vi "步进电机 - MO1.vi"() -> ()   [LabVIEW 2026, in "UI-步进.lvlib"]
doc: "本范例执行串口读写操作。串口设置的参数必须匹配连接仪器或设备的参数。“VISA配置串口”VI可设置配置参数。前面板显示的控件可用于配置基本参数，如波特率、数据位和校验。VI会将VISA资源名称传递至其他VI以便执行相关操作。“VISA写入”函数将发送一个命令至串行设备，“VISA读取”函数将返回基于该命令的数据。“VISA关闭”函数可关闭该串行设备的引用。关闭引用十分重要，否则可能导致无法通过该端口进行进一步通信。"
uses:
  Data ColndSave/Supports/Time and Data.ctl
  Supports/Sample Settings.ctl
  Supports/Repeat Steps.ctl
  <userlib>/_NEVSTOP/Communicable State Machine(CSM)/_Polymophic/CSM - Filter Duplicated Lines.vi
  b0ea00e1-49fa-42d0-971a-8e9f2f400525.vi
  20f4c7ca-4433-4752-8a12-caedff3309a5.vi
  a83f89c7-cc94-454f-8c22-caf8203e03ac.vi
  b673ad46-ecaf-4cfd-8bbb-6ae2088f5605.vi
  2e9f0e78-498b-41e3-86b1-c1255401f045.vi
  04a4e073-6b30-45d7-bb50-3b2b3a136a6d.vi
  2a4e068b-7d24-4fa7-ac03-c345972a0de1.vi
  44b8d297-727d-4724-bbbb-13bdb1641d5d.vi
  723f4e3d-5d0c-4f32-90dc-14f06c7549ca.vi
  796b8098-58f3-468a-8e00-fd722edcd372.vi
  f0ef90a9-37fd-4693-8a17-3839f28c21af.vi
  f65ec2b2-16c2-4de3-b539-835afd05168c.vi
  fd098784-0da8-4741-84dc-d815f177a802.vi
  <userlib>/_NEVSTOP/Communicable State Machine(CSM)/_Polymophic/CSM - Replace Marks in Messages.vi
  990eb54c-669a-44f1-af6b-0d611d3b61bb.vi
  2b2daabb-4cfa-4505-9e37-d62c08413a28.vi
  9c881153-a381-4589-a185-2ba02b3623cc.vi
  a1f5b737-46a0-46ad-8ba4-fb05ffa8a237.vi
  d5c603ec-7b80-4271-a83a-f9475fd1a065.vi
  c59def73-e1a7-4980-a83b-4e794f8740d4.vi
  95a76b64-0183-4b9d-a020-bf71b96b4595.vi
  12ea21cb-d699-47f4-8962-41d5d90be2ef.vi
  666677ec-4a5d-482c-b398-180d4b47e7ed.vi
  494b3fb5-273a-41a7-af20-8ee63da9d16f.vi
  0af2ad88-edd2-4f06-96cf-8fa513af6a10.vi
  2532b81a-ef6f-4dde-8bfe-c4d2e445e585.vi
  41f7d585-ae95-49ce-8fbc-6366eab20bab.vi
  57b87adc-c73b-462d-8ae1-05c1c70c80b4.vi
  b9a08e84-7226-4261-ac85-d69acd1971d6.vi
  <userlib>/_NEVSTOP/Communicable State Machine(CSM)/AdvanceAPI/CSM - Compact Multiple States.vi
  <userlib>/_NEVSTOP/Communicable State Machine(CSM)/AdvanceAPI/CSM - Break Down Multiple States String.vi
  <userlib>/_NEVSTOP/Communicable State Machine(CSM)/_Shared/Remove Comments from Single-line.vi
  <userlib>/_NEVSTOP/Communicable State Machine(CSM)/_Shared/Split Single-line Message.vi
  <userlib>/_NEVSTOP/Communicable State Machine(CSM)/_Shared/Trim Single-line Text.vi
  <userlib>/_NEVSTOP/Communicable State Machine(CSM)/AdvanceAPI/CSM - Revert Arguments-Safe String.vi
  <userlib>/_NEVSTOP/Communicable State Machine(CSM)/AdvanceAPI/CSM - Make String Arguments Safe.vi
  723f4e3d-5d0c-4f32-90dc-14f06c7549ca.vi/99de0c97-112a-4c86-9094-c187659127e1.vi
  <userlib>/_NEVSTOP/Communicable State Machine(CSM)/Utility/Build Error Cluster.vi
  796b8098-58f3-468a-8e00-fd722edcd372.vi/99de0c97-112a-4c86-9094-c187659127e1.vi
  f65ec2b2-16c2-4de3-b539-835afd05168c.vi/99de0c97-112a-4c86-9094-c187659127e1.vi
  fd098784-0da8-4741-84dc-d815f177a802.vi/99de0c97-112a-4c86-9094-c187659127e1.vi
  2532b81a-ef6f-4dde-8bfe-c4d2e445e585.vi/b09b9099-6be0-413b-8afc-4908471460c3.vi
  <userlib>/_NEVSTOP/Communicable State Machine(CSM)/addons/INI-Static-Variable-Support/_Support/FlagInstance-CSMINIVariable.vi
  b9a08e84-7226-4261-ac85-d69acd1971d6.vi/99de0c97-112a-4c86-9094-c187659127e1.vi
  <vilib>/Utility/error.llb/Trim Whitespace.vi
  <vilib>/Utility/error.llb/Trim Whitespace (string).vi
  <userlib>/_NEVSTOP/Communicable State Machine(CSM)/AdvanceAPI/CSM - Keywords.vi
  <userlib>/_NEVSTOP/Communicable State Machine(CSM)/_Support/ChangeFlag/ChangeFlag-Read.vi
  <vilib>/Utility/error.llb/Trim Whitespace One-Sided.vi
  <userlib>/_NEVSTOP/Communicable State Machine(CSM)/addons/INI-Static-Variable-Support/_Support/instances/_CSM - Read File Logger Configuration - v1.0.vi
  <vilib>/Utility/Data Type/Get Type Information.vi
  <userlib>/_NEVSTOP/Communicable State Machine(CSM)/addons/API-String-Arugments-Support/_Support/Data To SingleElementsArray_csm.vi
  <userlib>/_NEVSTOP/Communicable State Machine(CSM)/addons/API-String-Arugments-Support/_Support/Data To API String Arguments.vi
  <userlib>/_NEVSTOP/Communicable State Machine(CSM)/addons/INI-Static-Variable-Support/_Support/Parse Used Session and Name.vi
  <userlib>/_NEVSTOP/Communicable State Machine(CSM)/addons/INI-Static-Variable-Support/_Support/INI-FGV(lvlibp).vi
  <userlib>/_NEVSTOP/Communicable State Machine(CSM)/addons/INI-Static-Variable-Support/_Support/Populate String with INI Variable.vi
  <userlib>/_NEVSTOP/Communicable State Machine(CSM)/addons/API-String-Arugments-Support/_Support/Convert API String Arguments to Data(variant).vi
  <userlib>/_NEVSTOP/Communicable State Machine(CSM)/addons/API-String-Arugments-Support/_Support/SingleElementsArray To Data_csm.vi
  <userlib>/_NEVSTOP/Communicable State Machine(CSM)/addons/MassData-Parameter/_support/FGV-MassData(lvlibp).vi
  <vilib>/Instr/_visa.llb/VISA Configure Serial Port (Instr).vi
  <userlib>/_NEVSTOP/Communicable State Machine(CSM)/_Support/ChangeFlag/ChangeFlagDB.vi
  <userlib>/_NEVSTOP/Communicable State Machine(CSM)/Communicable State Machine.lvlib
  <userlib>/_NEVSTOP/Communicable State Machine(CSM)/addons/INI-Static-Variable-Support/INI-Static-Variable-Support.lvlib
  <userlib>/_NEVSTOP/Communicable State Machine(CSM)/addons/MassData-Parameter/CSM MassData Parameter Support.lvlib
  <userlib>/_NEVSTOP/Communicable State Machine(CSM)/addons/Watchdog/CSM Watchdog.lvlib
  <userlib>/_NEVSTOP/Communicable State Machine(CSM)/addons/Logger/CSM File Logger.lvlib
  Logging/Logging.lvlib
  Acquisition/Acquisition.lvlib
  Data ColndSave/Data Collection and Save.lvlib
  Repeat/Repeat.lvlib
panel:
  in  "步进电机显示":enum32{"步进电机", "循环功能", "联动功能", "Status"}(tab)
  in  "一键回原点":bool
  out "设置/读取报错":bool
  out "运行状态":bool
  in  "行程":i32 max=10 step=1
  in  "停止运行":bool
  in  "暂停":bool
  in  "速度(r/min)":i32=70 max=10 step=1
  in  "运行":bool
  in  "脱机使能":bool
  in  "加减速系数(0-10)":u8 max=10 step=1
  in  "运行单位":enum32{"脉冲", "圈数", "角度"}(radio)
  in  "电机开关":bool
  in  "步进电机串口":refnum<visa-resource-name>="COM4"
  out "步进电机位置":waveform(dbl)(graph)
  in  "运行方向":bool
  in  "CSM Name":string="MO1"
  in  "Interval(s)":dbl=0.5
  in  "电机循环":bool
  out "Error Occurred":errorcluster caption="步进电机-错误输出"
  in  "子程序？":bool
  out "State History":string
  in  "停止":bool
  # "电机连接"
  # "运行设置"
  # "基础功能"
  # "运行控制"
  # "状态显示"
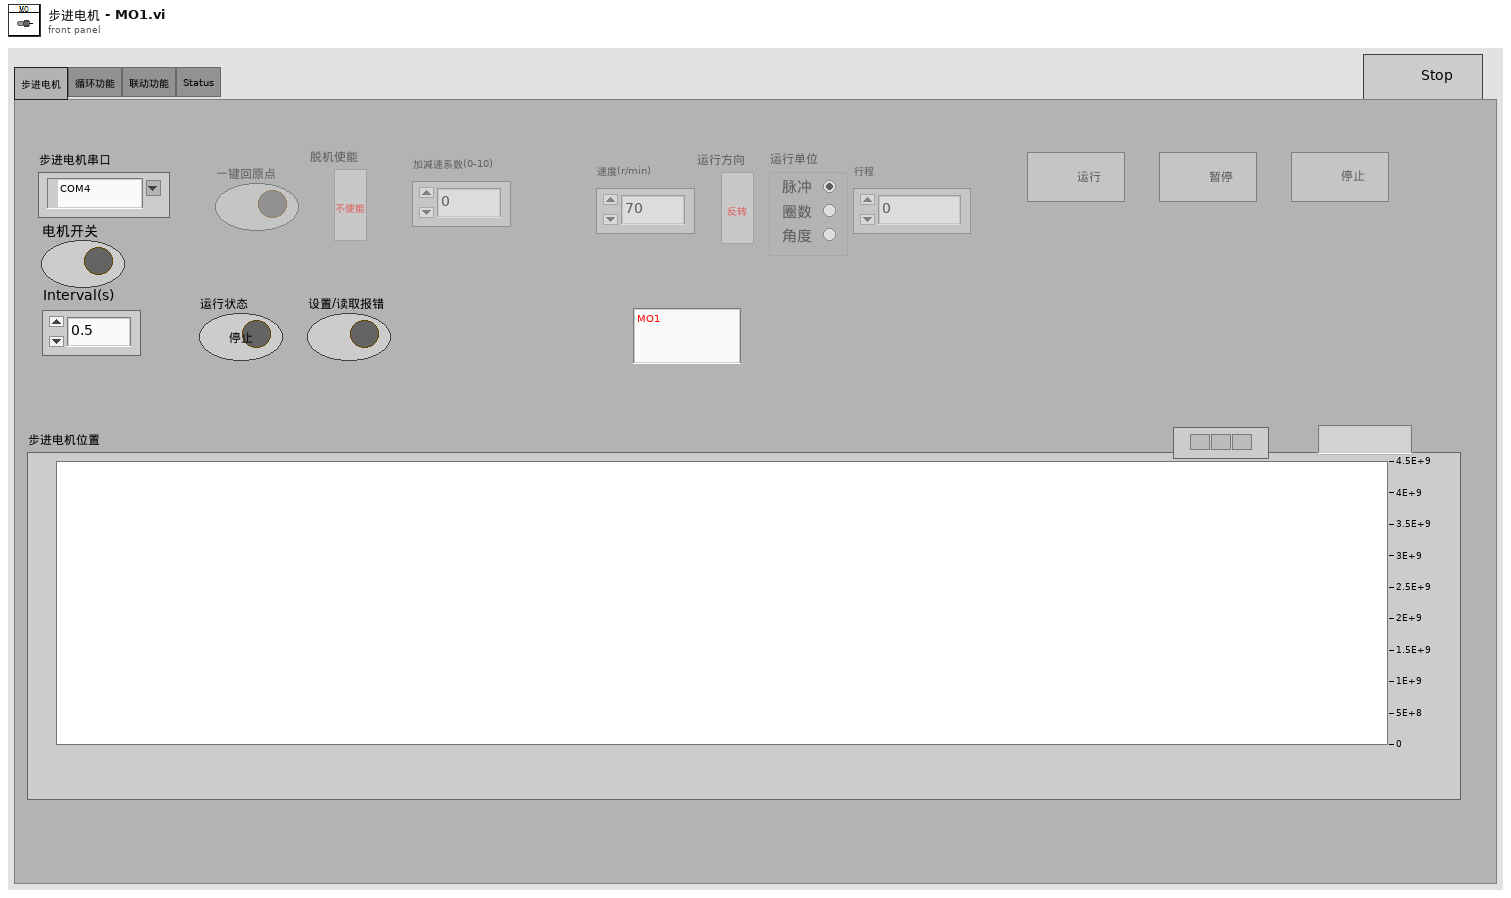
[diagram p1: front panel]
types:
  T1 = cluster{"Enable":bool, "Limit":cluster{"FileSize":i64, "FileNum":i32}, "Timestamp.Format":string, "AutoExit":bool}
  T2 = enum32{"Invalid", "Standard", "Closed", "Hidden", "Minimized", "Maximized"}
  T3 = enum32{"invalid app kind", "Development System", "Run Time System", "Student Edition", "Embedded LabVIEW", "Evaluation", "Custom"}
  T4 = cluster{"波特率":u32, "数据位":u16, "校验":enum16{"None", "Odd", "Even", "Mark", "Space"}, "停止位":u16, "流控制":u16}
  T5 = typedef "Communicable State Machine.lvlib/_CSM_Response Source Message.ctl" = cluster{"‘State":string, "’Arguments":string, "’Error":errorcluster}
  T6 = cluster{"Current VI Reference":refnum<vi>, "Close Panel on Exit?":bool}
  T7 = typedef "UI-步进.lvlib/Sample Settings.ctl" = cluster{"USB Port":refnum<visa-resource-name>, "采集间隔(s)":dbl, "位置":i32, "速度(r/min)":i32}
  T8 = typedef "Data Collection and Save.lvlib/Time and Data.ctl" = cluster{"采集时间":timestamp, "Data":dbl[]}
  T9 = cluster{"Core":cluster{"Current VI Reference":refnum<vi>, "Close Panel on Exit?":bool}, "Device Info":T7, "Time and Data":T8, "子程序？":bool, "Device Status":cluster{"方向":bool, "行程":i32, "单位地址":u8}}
  T10 = enum8{"Enabled", "Disabled", "Disabled and Grayed Out"}
  T11 = typedef "UI-步进.lvlib/Repeat Steps.ctl" = cluster{"行程":i32, "周期":i32, "进度":dbl, "光谱测量拿起":bool, "运行方向":bool}[]
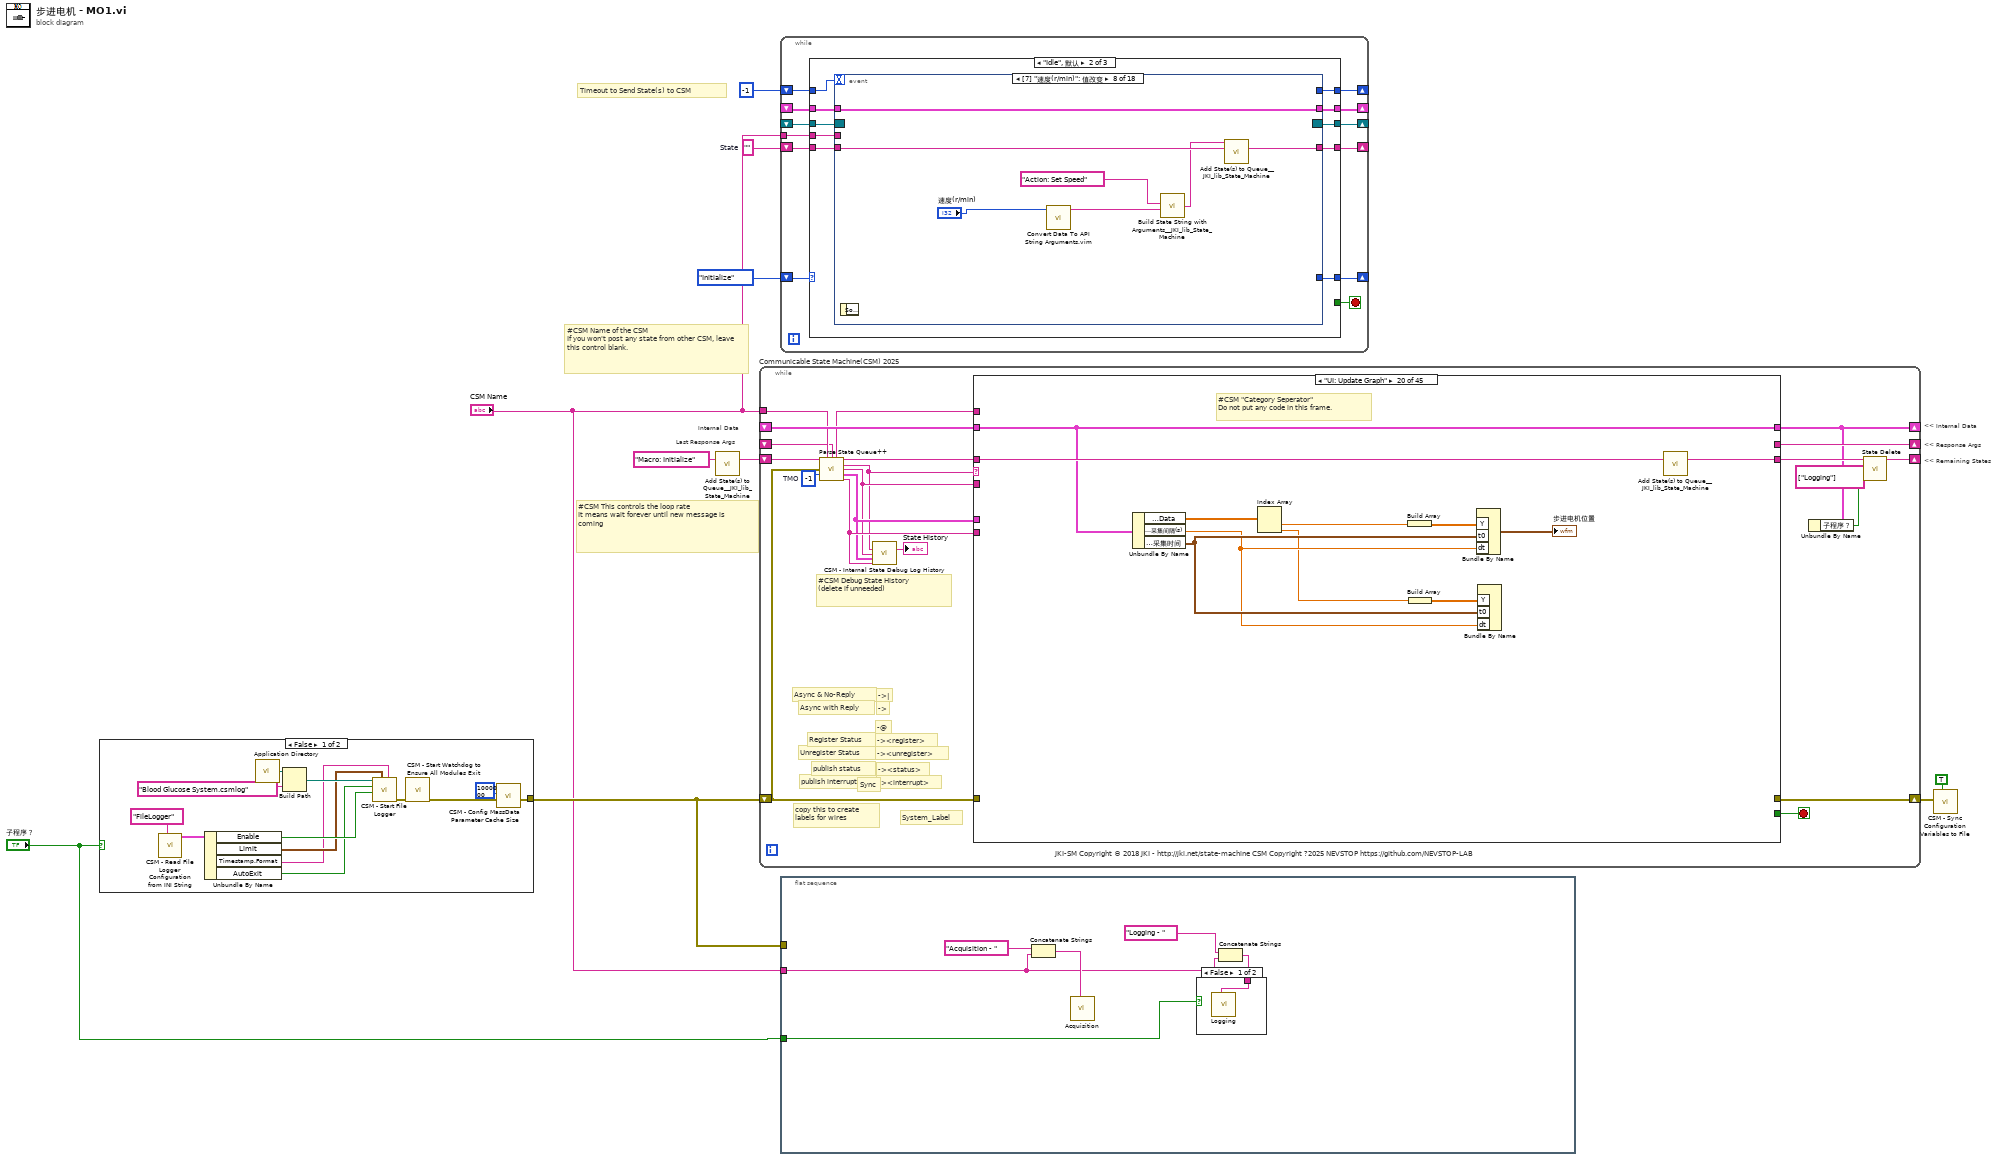
[diagram p0: block diagram]
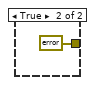
[diagram p2: hidden frame]
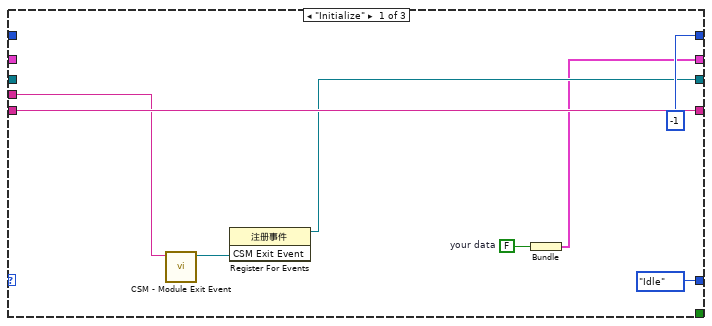
[diagram p4: hidden frame]
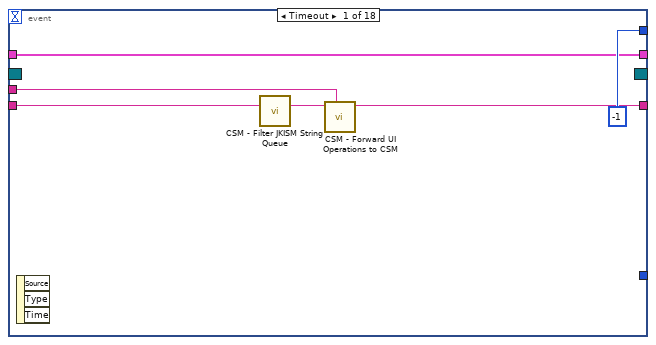
[diagram p5: hidden frame]
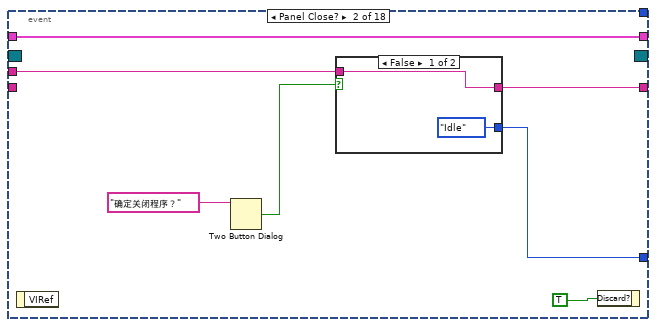
[diagram p6: hidden frame]
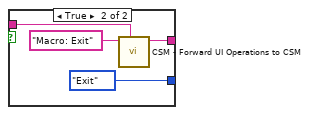
[diagram p7: hidden frame]
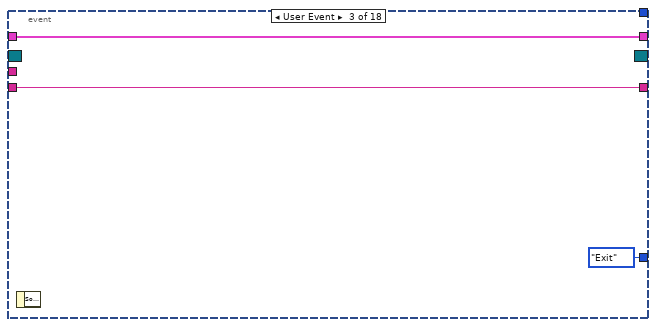
[diagram p8: hidden frame]
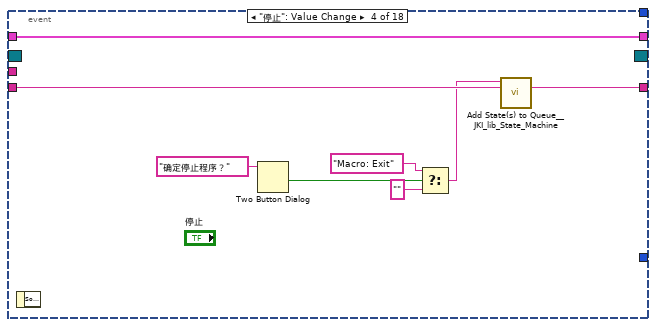
[diagram p9: hidden frame]
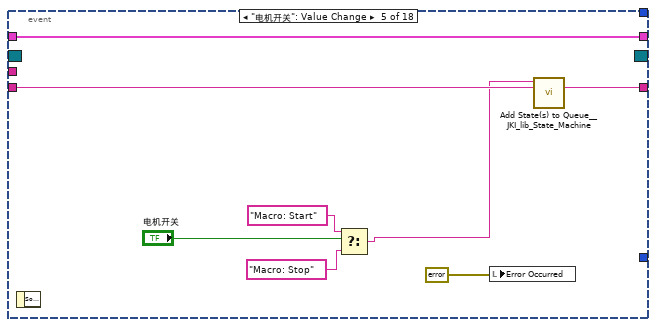
[diagram p10: hidden frame]
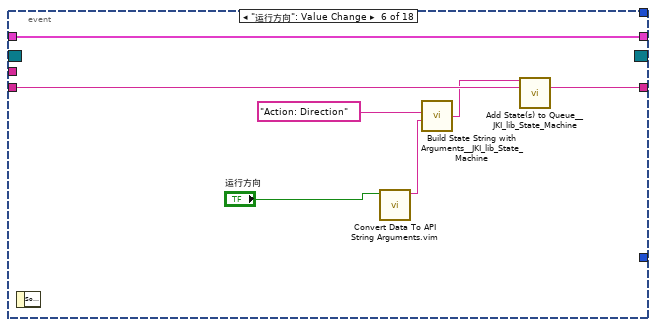
[diagram p11: hidden frame]
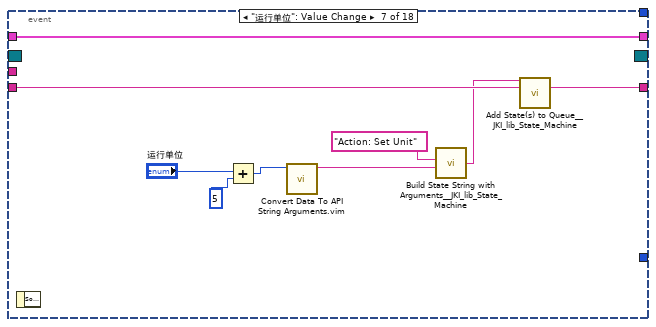
[diagram p12: hidden frame]
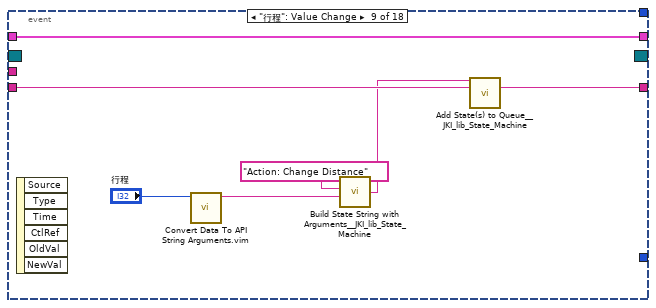
[diagram p13: hidden frame]
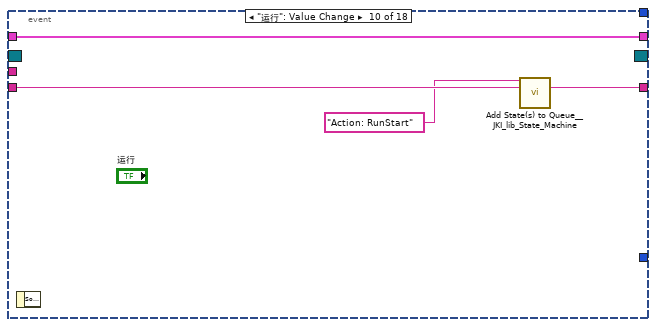
[diagram p14: hidden frame]
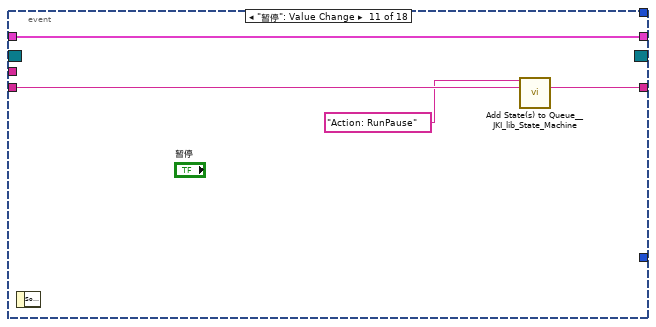
[diagram p15: hidden frame]
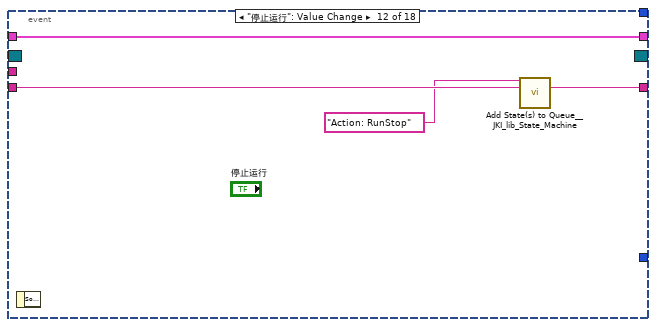
[diagram p16: hidden frame]
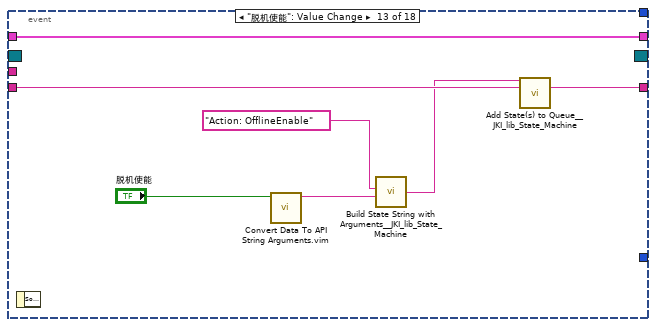
[diagram p17: hidden frame]
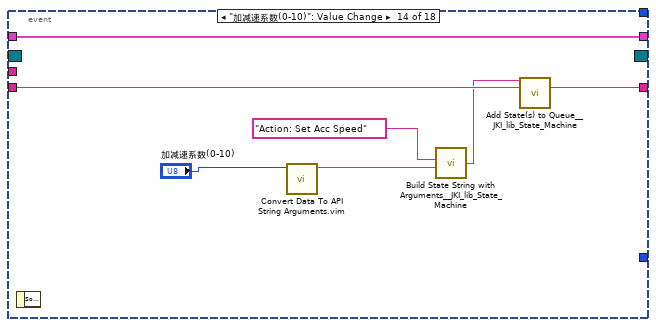
[diagram p18: hidden frame]
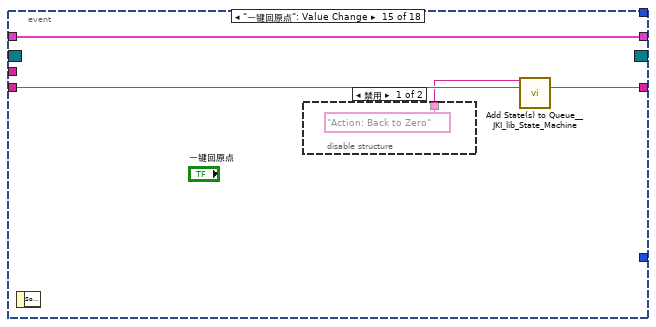
[diagram p19: hidden frame]
diagram:
  w9 = ""  # State
  # "Timeout to Send State(s) to CSM"
  # "Last Response Args"
  # "Internal Data"
  # "#CSM Name of the CSM\nIf you won't post any state from other CSM, leave this control blank."
  # "#CSM This controls the loop rate\nIt means wait forever until new message is coming"
  # "<< Internal Data"
  # "<< Response Args"
  # "<< Remaining States"
  n1 = case shown="False" "子程序？" {
    tunnel: [w11 errorcluster {"status"=FALSE, "code"=0, "source"=""} ("Error out")] -> w5
    frame False {
      n2 = call-poly <userlib>:"CSM - Read File Logger Configuration from INI String.vi"("Section Name(\"FileLogger\")"="FileLogger" ("Section Name(\"\" as Default)")) -> ("FileLogger Configuration-v1"=w18:T1)  [unwired: 7 in, 1 out]
      n3 = Unbundle By Name(w18) -> ("Enable"=w17:bool, "Limit"=w16:cluster{"FileSize":i64, "FileNum":i32}, "Timestamp.Format"=w14:string, "AutoExit"=w15:bool)
      n4 = call <vilib>:"Application Directory.vi"() -> ("Application Directory"=w23:path)
      n5 = Build Path(base path=w23, name or relative path="Blood Glucose System.csmlog") -> (appended path=w21:path)
      n6 = call <userlib>:"CSM - Start File Logger.vi"("Timestamp Format"=w14, "Log Limit"=w16, "Watchdog? (T)"=w17, "Exit When All Module Exist? (F)"=w15, "Log File Path"=w21) -> ("error out"=w20:errorcluster)  [unwired: 4 in, 2 out]
      n7 = call <userlib>:"CSM - Start Watchdog to Ensure All Modules Exit.vi"("error in (no error)"=w20) -> ("error out"=w12:errorcluster)  [unwired: 10 in]
      n8 = call <userlib>:"CSM - Config MassData Parameter Cache Size.vi"("Error in"=w12, "Size (50M)"=1000000 ("size(1M)")) -> ("Error out"=w11:errorcluster)  [unwired: 9 in]
    }
    frame True {
    }
  }
  n9 = call <vilib>:"Add State(s) to Queue__JKI_lib_State_Machine.vi"("State(s) in (\"\")"="Macro: Initialize" ("Init State(\"Macro: Initialize\")")) -> ("States Out"=w6:string)  [unwired: 14 in]
  n10 = while "Communicable State Machine(CSM) 2025" {
    shift-right: [w26] -> _
    shift-left: _ -> [w41]
    shift-right: [w43] -> w3
    shift-left: w5 -> [w31]
    shift-right: [w28] -> _
    shift-left: w6 -> [w44]
    tunnel: "CSM Name" -> [w38]
    shift-right: [w39] -> _
    shift-left: _ -> [w33]
    stop <- w42 stop-if-true
    w40 = -1  # TMO
    # "#CSM Debug State History\n(delete if unneeded)"
    # "-><interrupt>"
    # "-><status>"
    # "-><unregister>"
    # "-><register>"
    # "-@"
    # "->"
    # "->|"
    # "publish interrupt"
    # "publish status"
    # "Unregister Status"
    # "Register Status"
    # "Sync"
    # "Async with Reply"
    # "Async & No-Reply"
    # "JKI-SM Copyright © 2018 JKI - http://jki.net/state-machine CSM Copyright ?2025 NEVSTOP https://github.com/NEVSTOP-LAB"
    # "copy this to create labels for wires"
    # "System_Label"
    n11 = call <userlib>:"Parse State Queue++.vi"("State Queue"=w44, "Name (\"\" to Use UUID)"=w38, "Response Arguments"=w33, "Previous Error"=w31, "Dequeue (1 ms)"=w40) -> ("Name Used"=w32:string, "Remaining States"=w45:string, "Current State"=w34:string, "Arguments"=w35:string, "Additional Information"=w36:T5, "Source CSM"=w37:string)  [unwired: 5 in]
    n12 = call <userlib>:"CSM - Internal State Debug Log History.vi"("State"=w34, "Arguments (\"\")"=w35, ">> Response Source Message >>"=w36, "Source (\"\")"=w37) -> ("Debug Log"=→"State History":string)  [unwired: 11 in]
    n13 = case shown="\"UI: Update Graph\"" w34 {
      selector: w34 -> [_ _ _ w56 _ _ _ _ _ _ _ _ _ _ _ _ _ _ _ _ _ _ _ _ _ _ _ _ _ _ _ _ _ _ _ _ _ _ _ _ _ _ _ _ _]
      tunnel: w45 -> [w46 w49 w52 w60 w65 w71 w96 w102 w108 w118 w125 w137 w141 w144 w161 w168 w180 w183 w198 w209 w212 w218 w239 w264 w280 w285 w291 w294 w304 w319 w326 w340 w373 w383 w393 w409 w422 w424 w435 w442 w444 w458 w473 w482 w489]
      tunnel: w35 -> [_ _ _ _ _ w70 w92 w99 w105 w112 _ _ _ _ _ w166 _ _ _ _ _ _ _ _ _ _ _ _ w301 w318 w331 w339 _ _ _ w401 w414 _ w431 w441 _ _ w470 _ _]
      tunnel: w41 -> [w47 w48 w50 w58 w64 w76 w94 w100 w106 w116 w124 w131 w139 w142 _ w164 w175 w181 w184 w207 w210 w216 w220 w261 w275 w283 w289 w296 w306 w316 w324 w347 w358 w375 w385 w402 w415 w426 w428 w439 w446 w460 w475 w484 w491]
      tunnel: [_ _ _ w53 w66 errorcluster {"status"=FALSE, "code"=0, "source"=""} ("error out") w89 w97 w103 w119 _ _ _ _ _ _ w176 _ _ _ _ _ w231 w271 _ w282 _ _ w313 _ w336 w351 w360 w377 w387 w404 w417 _ _ _ w447 w461 w476 w485 w492] -> w43
      tunnel: w31 -> [_ _ _ w54 w66 w74 w90 w98 w104 _ _ _ _ _ _ _ w177 _ _ _ _ _ w231 w271 _ w282 _ _ w313 _ w336 w351 w361 w378 w388 w405 w418 _ _ _ w447 w461 w476 w485 w492]
      tunnel: [w46 w49 w51 w59 w65 w72 w95 w101 w107 w117 w125 w136 w140 w143 w160 w167 w179 w182 w197 w208 w211 w217 w238 w265 w279 w285 w290 w295 w305 w320 w327 w341 w374 w384 w394 w410 w423 w425 w436 w443 w445 w459 w474 w483 w490] -> w29
      tunnel: [_ _ _ _ _ _ TRUE _ _ _ _ _ TRUE _ _ _ _ _ _ _ _ _ _ _ _ _ _ _ _ _ _ _ _ _ _ _ _ _ _ _ _ _ _ _ _] -> w42
      tunnel: [w47 w48 w50 w58 w64 w76 w94 w100 w106 w115 w124 w135 w139 w142 w159 w163 w175 w181 w184 w207 w210 w216 w234 w260 w275 w283 w289 w296 w303 w314 w323 w346 w357 w375 w385 w402 w415 w426 w427 w438 w446 w460 w475 w484 w491] -> w26
      tunnel: w37 -> [_ _ _ _ _ w69 _ _ _ w113 _ _ _ _ _ _ _ _ _ _ _ _ _ _ _ _ _ _ _ _ _ _ _ _ _ _ _ _ _ _ _ _ _ _ _]
      tunnel: w36 -> [_ _ _ _ _ w68 _ _ _ w114 _ _ _ _ _ _ _ _ _ _ _ _ _ _ _ _ _ _ _ _ _ _ _ _ _ _ _ _ _ _ _ _ _ _ _]
      tunnel: [_ _ _ "" w61 _ _ _ _ _ _ _ _ _ _ _ _ _ _ _ _ _ _ _ _ _ _ _ _ _ _ _ _ _ _ _ _ _ _ _ _ _ _ _ _] -> w39
      tunnel: w32 -> [_ _ _ w55 _ _ w91 _ _ _ _ _ _ _ w145 _ w171 _ _ _ _ w214 w235 _ w277 _ w287 _ _ _ _ _ w352 _ _ _ _ _ w433 _ _ w450 _ _ _]
      frame "", "Idle" {
        # "#CSM \"Idle/Event Handler\"\nexecutes when the state queue is empty"
      }
      frame "CSM Documentation" {
        # "#CSM State Syntax\n\n// Comment line, all text to the right of “//” will be ignored\n// Local Message Example\nDoSth: DoA >> Arguments\n\n// Sync Call Example\nAPI: xxxx >> Arguments -@ TargetModule\n\n// Async Call Example\nAPI: xxxx >> Arguments -> TargetModule\n\n// Async Call without Reply Example\nAPI: xxxx >> Arguments ->| TargetModule\n\n// Broadcast normal status:\nStatus >> StatusArguments  -><status>\n\n// Broadcast Interrupt status:\nInterrupt >> StatusArguments  -><interrupt>\n\n// Register Source Module's status to Handler Module\nStatus@Source Module >> Handler Module@Handler Module -><register>\n\n// Unegister Source Module's status\nStatus@Source Module >> Handler Module -><unregister>"
        # "#CSM README FIRST\n\nCommunicable State Machine(CSM) is a LabVIEW application framework that builds upon JKI State Machine(JKISM). It follows the pattern of JKISM and extends the keywords to describe message communication between modules, including concepts such as Sync-Message, Async-Message, Subscription/Unsubscription of status - essential elements for creating reusable code modules. For more information, please visit the CSM wiki: https://nevstop-lab.github.io/CSM-Wiki/\n\nFor instructions on JKI State Machine, visit: \n    http://jki.net/state-machine/\nFor information about CSM, visit: \n    https://github.com/NEVSTOP-LAB"
        # "#CSM \"Documentation\"\nCase for holding CSM Documenation"
      }
      frame "---------- Core ----------" {
        # "#CSM \"Category Seperator\"\nDo not put any code in this frame."
        n14 = call <vilib>:"Add State(s) to Queue__JKI_lib_State_Machine.vi"("State(s) in (\"\")"=w52) -> ("States Out"=w51:string)  [unwired: 14 in]
      }
      frame Default {
        # "#CSM \"Default\"\nthis is used to capture unhandled states and typos"
        n15 = call <userlib>:"CSM Unhandled State Error.vi"("error in (no error)"=w54, "Undefined State"=w56, "CSM Name"=w55) -> ("error out"=w53:errorcluster)  [unwired: 8 in]
        n16 = call <vilib>:"Add State(s) to Queue__JKI_lib_State_Machine.vi"("State(s) in (\"\")"=w60) -> ("States Out"=w59:string)  [unwired: 14 in]
      }
      frame "VI Reference" {
        n17 = Unbundle By Name(w64) -> ("Core"=w63:T6)
        n18 = Unbundle By Name(w63) -> ("Current VI Reference"=w62:refnum<vi>)
        n19 = call <userlib>:"CSM - Convert Data to HexStr.vi"("Variant"=w62) -> ("HEX String (0-9,A-F)"=w61:string)  [unwired: 8 in]
      }
      frame "Error Handler" {
        # "#CSM \"Error Handler\"\nYou can also output any states to clean-up after errors occur"
        # "Clear error"
        n20 = case shown="错误" w74 {
          selector: w74 -> [_ w83]
          tunnel: [w81 w85] -> w73
          tunnel: w71 -> [w81 w84]
          tunnel: w70 -> [w80 _]
          tunnel: w69 -> [_ _]
          tunnel: w68 -> [_ _]
          tunnel: [w78 w83] -> w67
          frame No Error {
            n21 = call <userlib>:"CSM - Convert Argument to Error.vi"("Argument"=w80) -> ("Error"=w79:errorcluster)  [unwired: 4 in]
            n22 = flat-sequence {
              tunnel: w79 -> [w82]
              tunnel: [w82] -> w78
              frame #0 {
              }
            }
          }
          frame Error {
            # "#CSM Internal Error Handler Case \nIf any error Occurred, \"Error Occurred\" \nstatus update will be broadcasted to system.\nParameter is Error Cluster."
            n23 = call <userlib>:"CSM - Convert Error to Argument.vi"("Error"=w83) -> ("Argument"=w87:string)  [unwired: 4 in]
            n24 = call <vilib>:"Build State String with Arguments__JKI_lib_State_Machine.vi"("Arguments (\"\")"=w87, "State"="Error Occurred" ("Status with Arguments")) -> ("State with Arguments"=w86:string)  [unwired: 4 in]
            n25 = call <userlib>:"CSM - Broadcast Status Change.vi"("Status With Arguments"=w86, "State Queue"=w84) -> ("Remaining States"=w85:string)  [unwired: 13 in]
          }
        }
        "Error Occurred" <- w67
        n26 = call <vilib>:"Add State(s) to Queue__JKI_lib_State_Machine.vi"("State(s) in Front (\"\")"="// Post Error States", "State(s) in (\"\")"=w73) -> ("States Out"=w72:string)  [unwired: 13 in]
      }
      frame "Critical Error" {
        # "#CSM \"Critical Error\"\nWhen any un-recoverable error occurs, CSM goes into this case."
        # "#CSM Stop in Critical Error\nWhen Critical Error occurs, Stop the loop immediately. Do NOT change this unless you fully understand the impact."
        n27 = call <userlib>:"CSM Critical Error.vi"("error in (no error)"=w90, "Arugments (As Reason)"=w92, "CSM Name"=w91) -> ("error out"=w89:errorcluster)  [unwired: 8 in]
        n28 = call <vilib>:"Add State(s) to Queue__JKI_lib_State_Machine.vi"("State(s) in (\"\")"=w96) -> ("States Out"=w95:string)  [unwired: 14 in]
      }
      frame "Target Timeout Error" {
        # "#CSM \"Target Timeout Error\"\nWhen This CSM could not get the sync-call response in time, This CSM goes into this case."
        n29 = call <userlib>:"CSM Target Timeout Error.vi"("error in (no error)"=w98, "Arguments (As CSM Name)"=w99) -> ("error out"=w97:errorcluster)  [unwired: 9 in]
        n30 = call <vilib>:"Add State(s) to Queue__JKI_lib_State_Machine.vi"("State(s) in (\"\")"=w102) -> ("States Out"=w101:string)  [unwired: 14 in]
      }
      frame "Target Error" {
        # "#CSM \"Target Error\"\nWhen This CSM try to communicate with an un-existed CSM, This CSM goes into this case."
        n31 = call <userlib>:"CSM Target Error.vi"("error in (no error)"=w104, "Arguments (As CSM Name)"=w105) -> ("error out"=w103:errorcluster)  [unwired: 9 in]
        n32 = call <vilib>:"Add State(s) to Queue__JKI_lib_State_Machine.vi"("State(s) in (\"\")"=w108) -> ("States Out"=w107:string)  [unwired: 14 in]
      }
      frame "Async Response", "Response" {
        n33 = Unbundle(w114) -> ("‘State"=w111:string, "’Arguments"=w110:string, "’Error"=w109:errorcluster)
        n34 = case shown="默认" w111 {
          tunnel: [w120] -> w117
          tunnel: w118 -> [w121]
          tunnel: [w123] -> w115
          tunnel: w116 -> [w123]
          tunnel: [w122] -> w119
          tunnel: w109 -> [w122]
          tunnel: w113 -> [_]
          tunnel: w112 -> [_]
          tunnel: w110 -> [_]
          frame 默认 {
            # "#CSM \"Async Response\"\nHandle Async-call Response (\"Async Response\" for ->)"
            # "#CSM \"Response\"\nHandle Sync-call Response (\"Response\" for -@)"
            # "#CSM Response Comments\nAfter Message is executed, CSM goes to this state for receive the response.\n    For Async Message(->), \"Async Response\" is used. This CSM will goes to \"Async Message Posted\" immediately and receive the \"Async Response\" after the callee finishes the message.\n    For Sync Message(@),  This CSM will wait until the message is done and immediately goes to \"Response\""
            n35 = call <vilib>:"Add State(s) to Queue__JKI_lib_State_Machine.vi"("State(s) in (\"\")"=w121) -> ("States Out"=w120:string)  [unwired: 14 in]
          }
        }
      }
      frame "Async Message Posted" {
        # "#CSM \"Async Message Posted\"\nAfter Async Message is posted (-> or ->| ), CSM goes to this state for post-action.\nYou can use Argument - State to tell which Async Message is called."
      }
      frame "Initialize Core Data" {
        # "#CSM \"Initialize Core Data\"\nThis is used to determine panel behavior on exit"
        # "originally closed?"
        # "exe?"
        # "If panel starts closed or is an EXE, then close it when we exit"
        n36 = property class="VI"() -> ("FP.State"=w128:T2)  [unwired: 2 in, 2 out]
        n37 = property class="App"() -> ("App.Kind"=w134:T3)  [unwired: 2 in, 2 out]
        n38 = control-ref of="Current VI Reference"() -> (w129:refnum<vi>)
        n39 = Equal?(x=w128, y=T2."Closed" ("Front Panel Window:State")) -> (x = y?=w126:bool)
        n40 = Equal?(x=w134, y=T3."Run Time System" ("Application:Kind")) -> (x = y?=w132:bool)
        n41 = Or(x=w126, y=w132) -> (x .or. y?=w130:bool)
        n42 = Bundle By Name(cluster=w131, "Core.Current VI Reference"=w129, "Core.Close Panel on Exit?"=w130) -> (w135:T9)
        n43 = call <vilib>:"Add State(s) to Queue__JKI_lib_State_Machine.vi"("State(s) in (\"\")"=w137) -> ("States Out"=w136:string)  [unwired: 14 in]
      }
      frame "Exit" {
        # "#CSM \"Exit\"\nCase for exiting the loop. No errors that occur here will be handled."
        n44 = call <vilib>:"Add State(s) to Queue__JKI_lib_State_Machine.vi"("State(s) in (\"\")"=w141) -> ("States Out"=w140:string)  [unwired: 14 in]
      }
      frame "---------- Data ----------" {
        # "#CSM \"Category Seperator\"\nDo not put any code in this frame."
        n45 = call <vilib>:"Add State(s) to Queue__JKI_lib_State_Machine.vi"("State(s) in (\"\")"=w144) -> ("States Out"=w143:string)  [unwired: 14 in]
      }
      frame "Data: Initialize" {
        w146 = cluster{"方向":bool, "行程":i32, "单位地址":u8} {"方向"=FALSE, "行程"=0, "单位地址"=0}  # Device Status
        w151 = T7 {"USB Port"="", "采集间隔(s)"=0.5, "位置"=0, "速度(r/min)"=70}  # Device Info
        w150 = FALSE ("结束")
        w156 = T8 {"采集时间"=timestamp(0 s since 1904-01-01), "Data"=[0.0, 0.0]}  # Time and Data
        w158 = T6 {"Current VI Reference"=refnum, "Close Panel on Exit?"=FALSE}  # Core
        # "#CSM \"Data: Initialize\"\nInitialize the shift-register data, here.\n(data names are defined by what you wire into the bundle function)"
        # "#CSM do not delete - used by framework"
        # "#CSM Add new data here."
        # "#CSM Data names and types of shift register data are defined by this bundle."
        n46 = local write "Error Occurred"(errorcluster {"status"=FALSE, "code"=0, "source"=""} ("Error Occurred")) -> ()
        n47 = local read "子程序？"() -> (w155:bool)
        n48 = call "CSM - Read Cluster Elements From Session.vim"("Section Name (\"\" as Default)"=w145, "Cluster"=w146) -> ("Cluster out"=w148:cluster{"方向":bool, "行程":i32, "单位地址":u8})  [unwired: 6 in, 1 out]
        n49 = call "CSM - Read Cluster Elements From Session.vim"("Section Name (\"\" as Default)"=w145, "Cluster"=w151) -> ("Cluster out"=w154:T7)  [unwired: 6 in, 1 out]
        n50 = Select(t=w148, s=TRUE, f=w146) -> (s? t:f=w147:cluster{"方向":bool, "行程":i32, "单位地址":u8})
        n51 = local write "电机开关"(w150) -> ()
        n52 = Select(t=w154, s=TRUE, f=w151) -> (s? t:f=w152:T7)
        n53 = local write "电机循环"(w150) -> ()
        n54 = Bundle("Core"=w158, "Device Info"=w152, "Time and Data"=w156, "子程序？"=w155, "Device Status"=w147) -> (w159:T9)  [unwired: 1 in]
        n55 = call <vilib>:"Add State(s) to Queue__JKI_lib_State_Machine.vi"("State(s) in (\"\")"=w161) -> ("States Out"=w160:string)  [unwired: 14 in]
        "运行状态" <- w150
        "设置/读取报错" <- w150
      }
      frame "Data: Update Indicators" {
        w165 = T8 {"采集时间"=timestamp(0 s since 1904-01-01), "Data"=[]}  # Time and Data
        n56 = call "CSM - Convert Argument to MassData.vim"("Type"=w165, "MassData Argument"=w166) -> ("Data"=w162:T8)  [unwired: 6 in, 1 out]
        n57 = in-place {
          in-place-border: w162 -> [w170]
          n58 = in-place-cluster #1(w164) -> ()  [unwired: 1 out]
          n59 = in-place-cluster #1("Time and Data"=w170) -> (w163:T9)
        }
        n60 = call <vilib>:"Add State(s) to Queue__JKI_lib_State_Machine.vi"("State(s) in Front (\"\")"="UI: Update Graph" ("State(s) in Front (\"\")"), "State(s) in (\"\")"=w168) -> ("States Out"=w167:string)  [unwired: 13 in]
      }
      frame "Data: Cleanup" {
        w173 = FALSE ("温度采集开关")
        # "#CSM \"Data: Cleanup\"\nCleanup any data and references, here.\n(this is called automatically, by the Macro: Exit)"
        n61 = Unbundle By Name(w175) -> ("Core.Current VI Reference"=w178:refnum<vi>, "Device Info"=w174:T7, "Device Status"=w172:cluster{"方向":bool, "行程":i32, "单位地址":u8})
        n62 = call "CSM - Write Configuration Variable.vim"("Section Name (\"\" as Default)"=w171, "Configuration"=w172) -> ()  [unwired: 6 in, 2 out]
        n63 = call "CSM - Write Configuration Variable.vim"("Section Name (\"\" as Default)"=w171, "Configuration"=w174) -> ()  [unwired: 6 in, 2 out]
        n64 = Close Reference(reference=w178, error in (no error)=w177) -> (error out=w176:errorcluster)
        n65 = local write "电机循环"(w173) -> ()
        n66 = local write "电机开关"(w173) -> ()
        n67 = call <vilib>:"Add State(s) to Queue__JKI_lib_State_Machine.vi"("State(s) in (\"\")"=w180) -> ("States Out"=w179:string)  [unwired: 14 in]
      }
      frame "---------- UI ----------" {
        # "#CSM \"Category Seperator\"\nDo not put any code in this frame."
        n68 = call <vilib>:"Add State(s) to Queue__JKI_lib_State_Machine.vi"("State(s) in (\"\")"=w183) -> ("States Out"=w182:string)  [unwired: 14 in]
      }
      frame "UI: Initialize" {
        w191 = T10."Disabled and Grayed Out" ("禁用")
        # "#CSM \"Category Seperator\"\nDo not put any code in this frame."
        n69 = Unbundle By Name(w184) -> ("Device Info.速度(r/min)"=w190:i32, "Device Info.USB Port"=w193:refnum<visa-resource-name>, "Device Info.采集间隔(s)"=w196:dbl, "Device Status.方向"=w185:bool, "Device Status.行程"=w186:i32, "Device Status.单位地址"=w188:u8, "子程序？"=w195:bool)
        n70 = Not(x=w195) -> (.not. x?=w194:bool)
        n71 = Subtract(x=w188, y=u8 5 ("寄存器地址")) -> (x-y=w187:u8)
        n72 = local write "速度(r/min)"(w190) -> ()
        n73 = local write "步进电机串口"(w193) -> ()
        n74 = local write "Interval(s)"(w196) -> ()
        n75 = local write "运行方向"(w185) -> ()
        n76 = property on="步进电机位置" class="WFChart (严格)"("History Data"=waveform(dbl)[] [] ("历史数据")) -> ()  [unwired: 2 in, 2 out]
        n77 = property on="停止" class="Bool"("Visible"=w194) -> ()  [unwired: 2 in, 2 out]
        n78 = local write "运行单位"(w187) -> ()
        n79 = local write "行程"(w186) -> ()
        n80 = property on="一键回原点" class="Bool"("DisabledEnum"=w191) -> ()  [unwired: 2 in, 2 out]
        n81 = property on="脱机使能" class="Bool (严格)"("DisabledEnum"=w191) -> ()  [unwired: 2 in, 2 out]
        n82 = property on="加减速系数(0-10)" class="DigNum (严格)"("DisabledEnum"=w191) -> ()  [unwired: 2 in, 2 out]
        n83 = property on="速度(r/min)" class="DigNum (严格)"("DisabledEnum"=w191) -> ()  [unwired: 2 in, 2 out]
        n84 = property on="运行方向" class="Bool (严格)"("DisabledEnum"=w191) -> ()  [unwired: 2 in, 2 out]
        n85 = property on="运行单位" class="RadioBtnsControl (严格)"("DisabledEnum"=w191) -> ()  [unwired: 2 in, 2 out]
        n86 = property on="行程" class="DigNum (严格)"("DisabledEnum"=w191) -> ()  [unwired: 2 in, 2 out]
        n87 = property on="运行" class="Bool"("DisabledEnum"=w191) -> ()  [unwired: 2 in, 2 out]
        n88 = property on="暂停" class="Bool"("DisabledEnum"=w191) -> ()  [unwired: 2 in, 2 out]
        n89 = property on="停止运行" class="Bool"("DisabledEnum"=w191) -> ()  [unwired: 2 in, 2 out]
        n90 = property on="电机循环" class="Bool (严格)"("DisabledEnum"=w191) -> ()  [unwired: 2 in, 2 out]
        n91 = call <vilib>:"Add State(s) to Queue__JKI_lib_State_Machine.vi"("State(s) in (\"\")"=w198) -> ("States Out"=w197:string)  [unwired: 14 in]
      }
      frame "UI: Update Graph" {
        # "#CSM \"Category Seperator\"\nDo not put any code in this frame."
        n92 = Unbundle By Name(w207) -> ("Time and Data.Data"=w204:dbl[], "Device Info.采集间隔(s)"=w201:dbl, "Time and Data.采集时间"=w202:timestamp)
        n93 = Index Array(array=w204) -> (element #1=w203:dbl, element #2=w200:dbl)  [unwired: 2 in]
        n94 = Build Array(w203) -> (w206:dbl[])
        n95 = Build Array(w200) -> (w205:dbl[])
        n96 = Bundle By Name("Y"=w206, "t0"=w202, "dt"=w201) -> (→"步进电机位置":waveform(dbl))  [unwired: 1 in]
        n97 = Bundle By Name("Y"=w205, "t0"=w202, "dt"=w201) -> ()  [unwired: 1 in, 1 out]
        n98 = call <vilib>:"Add State(s) to Queue__JKI_lib_State_Machine.vi"("State(s) in (\"\")"=w209) -> ("States Out"=w208:string)  [unwired: 14 in]
      }
      frame "---------- Macro ----------" {
        # "#CSM \"Category Seperator\"\nDo not put any code in this frame."
        n99 = call <vilib>:"Add State(s) to Queue__JKI_lib_State_Machine.vi"("State(s) in (\"\")"=w212) -> ("States Out"=w211:string)  [unwired: 14 in]
      }
      frame "Macro: Initialize" {
        w215 = "Data: Initialize\nInitialize Core Data\nUI: Initialize\n\n//Permanent registrations\nAcquired Data@Acquisition - <1> >> Data: Update Indicators -><register>\nAcquired Data@Acquisition - <1> >> API: Log@Logging - <1> -><register>\n\n//Error registrations\nError Occurred@Acquisition - <1> >> Error Handler -><register>\nError Occurred@Logging - <1> >> Error Handler -><register>\n\n//Dynamic registrations\n// 订阅/取消订阅\n//Status@SourceModule >> API@TargetModule -><register as interrupt>\n//UrgentEvent @SourceModule >> API@TargetModule -><register as status>\n\n\n\n//Launch Acquisition Module\n"  # Data: Initialize Initialize Core Data UI: Initialize  //Permanent registrations Acquired Data@Acquisition - <1> >> Data: Update Indicators -><register> Acquired Data@Acquisition - <1> >> API: Log@Logging - <1> -><register>  //Error registrations Error Occurred@Acquisition - <1> >> Error Handler -><register> Error Occurred@Logging - <1> >> Error Handler -><register>  //Dynamic registrations // 订阅/取消订阅 //Status@SourceModule >> API@TargetModule -><register as interrupt> //UrgentEvent @SourceModule >> API@TargetModule -><register as status>    //Launch Acquisition Module
        # "#CSM \"Macro: Initialize\"\nInitialization Macro (This is called once, when the VI starts)"
        n100 = call-poly <userlib>:"Build Message with Arguments++.vi"("States With Replace Token"=w215, "<1>"=w214) -> ("States"=w213:string)  [unwired: 13 in]
        n101 = call <vilib>:"Add State(s) to Queue__JKI_lib_State_Machine.vi"("State(s) in Front (\"\")"=w213, "State(s) in (\"\")"=w218) -> ("States Out"=w217:string)  [unwired: 13 in]
      }
      frame "Macro: Start" {
        w222 = T10."Enabled" ("禁用")
        n102 = Unbundle By Name(w220) -> ("Device Info.USB Port"=w219:refnum<visa-resource-name>)
        n103 = Unbundle By Name(T4 {"波特率"=9600, "数据位"=8, "校验"=enum."None", "停止位"=10, "流控制"=0} ("串口设置")) -> ("波特率"=w224:u32, "数据位"=w226:u16, "校验"=w227:enum16{"None", "Odd", "Even", "Mark", "Space"}, "停止位"=w228:u16, "流控制"=w229:u16)
        n104 = local write "电机开关"(TRUE ("温度采集开关")) -> ()
        n105 = call-poly "VISA Configure Serial Port"("VISA resource name"=w219, "baud rate (9600)"=w224, "data bits (8)"=w226, "parity (0:none)"=w227, "stop bits (10: 1 bit)"=w228, "flow control (0:none)"=w229) -> ("VISA resource name out"=w221:refnum<visa-resource-name>)  [unwired: 3 in, 6 out]
        n106 = Bundle By Name(cluster=w220, "Device Info.USB Port"=w221, "Device Info.位置"=0 ("Device Status.位置")) -> (w234:T9)
        n107 = Unbundle By Name(w234) -> ("Device Info"=w232:T7)
        n108 = property on="一键回原点" class="Bool"("DisabledEnum"=w222) -> ()  [unwired: 2 in, 2 out]
        n109 = property on="脱机使能" class="Bool (严格)"("DisabledEnum"=w222) -> ()  [unwired: 2 in, 2 out]
        n110 = property on="加减速系数(0-10)" class="DigNum (严格)"("DisabledEnum"=w222) -> ()  [unwired: 2 in, 2 out]
        n111 = property on="速度(r/min)" class="DigNum (严格)"("DisabledEnum"=w222) -> ()  [unwired: 2 in, 2 out]
        n112 = property on="运行方向" class="Bool (严格)"("DisabledEnum"=w222) -> ()  [unwired: 2 in, 2 out]
        n113 = property on="运行单位" class="RadioBtnsControl (严格)"("DisabledEnum"=w222) -> ()  [unwired: 2 in, 2 out]
        n114 = property on="行程" class="DigNum (严格)"("DisabledEnum"=w222) -> ()  [unwired: 2 in, 2 out]
        n115 = property on="运行" class="Bool"("DisabledEnum"=w222) -> ()  [unwired: 2 in, 2 out]
        n116 = property on="暂停" class="Bool"("DisabledEnum"=w222) -> ()  [unwired: 2 in, 2 out]
        n117 = property on="停止运行" class="Bool"("DisabledEnum"=w222) -> ()  [unwired: 2 in, 2 out]
        n118 = property on="电机循环" class="Bool (严格)"("DisabledEnum"=w222) -> ()  [unwired: 2 in, 2 out]
        n119 = call "Convert Data To API String Arguments.vim"("Data"=w232) -> ("API String"=w236:string)  [unwired: 7 in, 1 out]
        n120 = call-poly <userlib>:"Build Message with Arguments++.vi"("States With Replace Token"="Macro: Init\nAPI: Start >> <param> -@ Acquisition - <1>\nAPI: Start  -@ Logging - <1>" ("State"), "<param>"=w236, "<1>"=w235) -> ("States"=w230:string)  [unwired: 12 in]
        n121 = call <vilib>:"Add State(s) to Queue__JKI_lib_State_Machine.vi"("State(s) in Front (\"\")"=w230, "State(s) in (\"\")"=w239) -> ("States Out"=w238:string)  [unwired: 13 in]
      }
      frame "Macro: Init" {
        w250 = FALSE ("读/写")
        # "加减速系数"
        # "脱机使能"
        # "行程"
        # "速度"
        # "方向"
        n122 = Unbundle By Name(w261) -> ("Device Status.单位地址"=w247:u8, "Device Info.USB Port"=w274:refnum<visa-resource-name>)
        n123 = call "串口读写 - 步进电机 - MO1.vi"("寄存器地址"=u8 1, "错误输入（无错误）"=w271, "写/读"=w250, "VISA输入"=w274) -> ("错误输出"=w266:errorcluster, "读取设备(n)"=w270:i32, "报错"=w246:bool, "VISA输出"=w267:refnum<visa-resource-name>)  [unwired: 4 in]
        n124 = Number To Boolean Array(number=w270) -> (Boolean array=w273:bool[])
        n125 = Index Array(array=w273) -> (element=w269:bool)  [unwired: 1 in]
        n126 = local write "运行方向"(w269) -> ()
        n127 = call "串口读写 - 步进电机 - MO1.vi"("寄存器地址"=u8 4, "错误输入（无错误）"=w266, "写/读"=w250, "VISA输入"=w267) -> ("错误输出"=w262:errorcluster, "读取设备(n)"=w240:i32, "报错"=w244:bool, "VISA输出"=w263:refnum<visa-resource-name>)  [unwired: 4 in]
        n128 = local write "速度(r/min)"(w240) -> ()
        n129 = call "串口读写 - 步进电机 - MO1.vi"("寄存器地址"=w247, "错误输入（无错误）"=w262, "写/读"=w250, "VISA输入"=w263) -> ("错误输出"=w258:errorcluster, "读取设备(n)"=w248:i32, "报错"=w243:bool, "VISA输出"=w259:refnum<visa-resource-name>)  [unwired: 4 in]
        n130 = local write "行程"(w248) -> ()
        n131 = call "串口读写 - 步进电机 - MO1.vi"("寄存器地址"=u8 9, "错误输入（无错误）"=w258, "写/读"=w250, "VISA输入"=w259) -> ("错误输出"=w251:errorcluster, "读取设备(n)"=w255:i32, "报错"=w242:bool, "VISA输出"=w252:refnum<visa-resource-name>)  [unwired: 4 in]
        n132 = Number To Boolean Array(number=w255) -> (Boolean array=w256:bool[])
        n133 = Index Array(array=w256) -> (element=w254:bool)  [unwired: 1 in]
        n134 = local write "脱机使能"(w254) -> ()
        n135 = call "串口读写 - 步进电机 - MO1.vi"("寄存器地址"=u8 14, "错误输入（无错误）"=w251, "写/读"=w250, "VISA输入"=w252) -> ("读取设备(n)"=w249:i32, "报错"=w241:bool)  [unwired: 4 in, 2 out]
        n136 = local write "加减速系数(0-10)"(w249) -> ()
        n137 = Compound Arithmetic op=OR ("复合运算")(w246, w244, w243, w242, w241) -> (w245:bool)
        n138 = local write "设置/读取报错"(w245) -> ()
        n139 = Bundle By Name(cluster=w261, "Device Status.行程"=w248) -> (w260:T9)
        n140 = call <vilib>:"Add State(s) to Queue__JKI_lib_State_Machine.vi"("State(s) in (\"\")"=w264) -> ("States Out"=w265:string)  [unwired: 14 in]
      }
      frame "Macro: Stop" {
        # "#CSM \"Macro: Exit\"\nExit Macro (This is called once, when the VI exits)"
        n141 = call-poly <userlib>:"Build Message with Arguments++.vi"("States With Replace Token"="//Send Message to Other CSM Modules\nAPI: Stop -@ Acquisition - <1>\nAPI: Stop -@ Logging - <1>\n\nMacro: Close", "<1>"=w277) -> ("States"=w276:string)  [unwired: 13 in]
        n142 = call <vilib>:"Add State(s) to Queue__JKI_lib_State_Machine.vi"("State(s) in Front (\"\")"=w276, "State(s) in (\"\")"=w280) -> ("States Out"=w279:string)  [unwired: 13 in]
      }
      frame "Macro: Close" {
        n143 = Unbundle By Name(w283) -> ("Device Info.USB Port"=w284:refnum<visa-resource-name>)
        n144 = local write "电机开关"(FALSE ("电机开关")) -> ()
        n145 = VISA Close(VISA resource name=w284, error in (no error)=w282) -> ()  [unwired: 1 out]
      }
      frame "Macro: Exit" {
        w288 = "//Exit\nMacro: Exit-@Acquisition - <1>\nMacro: Exit-@Logging - <1>\n\n//Permanent unregistrations\nAcquired Data@Acquisition - <1> >> Data: Update Indicators -><unregister>\nAcquired Data@Acquisition - <1> >> API: Log@Logging - <1> -><unregister>\n\n//Permanent unregistrations\nError Occurred@Acquisition - <1> >> Error Handler -><unregister>\nError Occurred@Logging - <1> >> Error Handler -><unregister>\n\nData: Cleanup\nExit"  # //Exit Macro: Exit-@Acquisition - <1> Macro: Exit-@Logging - <1>  //Permanent unregistrations Acquired Data@Acquisition - <1> >> Data: Update Indicators -><unregister> Acquired Data@Acquisition - <1> >> API: Log@Logging - <1> -><unregister>  //Permanent unregistrations Error Occurred@Acquisition - <1> >> Error Handler -><unregister> Error Occurred@Logging - <1> >> Error Handler -><unregister>  Data: Cleanup Exit
        # "#CSM \"Macro: Exit\"\nExit Macro (This is called once, when the VI exits)"
        n146 = disable-structure shown="禁用" {
          frame Disabled {
            # "#NOTE\nHelper VI is equivalent to other case"
            n147 = call <userlib>:"CSM - Build Exit Messages of CSMs.vi"("State With Arguments (\"Macro: Exit“)"="Macro: Exit" ("State with Arguments(\"Macro: Exit“)"), "CSMs"=string[] ["AcquisitionTP1", "//LoggingTP1"]) -> ()  [unwired: 13 in, 1 out]
          }
          frame Enabled {
          }
        }
        n148 = call-poly <userlib>:"Build Message with Arguments++.vi"("States With Replace Token"=w288, "<1>"=w287) -> ("States"=w286:string)  [unwired: 13 in]
        n149 = call <vilib>:"Add State(s) to Queue__JKI_lib_State_Machine.vi"("State(s) in Front (\"\")"=w286, "State(s) in (\"\")"=w291) -> ("States Out"=w290:string)  [unwired: 13 in]
      }
      frame "---------- Action ----------" {
        # "#CSM \"Category Seperator\"\nDo not put any code in this frame."
        n150 = call <vilib>:"Add State(s) to Queue__JKI_lib_State_Machine.vi"("State(s) in (\"\")"=w294) -> ("States Out"=w295:string)  [unwired: 14 in]
      }
      frame "Action: Direction" {
        # "方向"
        n151 = Unbundle By Name(w306) -> ("Device Info.USB Port"=w308:refnum<visa-resource-name>)
        n152 = call "Convert API String Arguments to Data.vim"("Reference Type"=FALSE, "API String"=w301) -> ("Data"=w297:bool)  [unwired: 6 in, 1 out]
        n153 = Boolean To (0,1)(Boolean=w297) -> (0, 1=w300:i16)
        n154 = To Long Integer(number=w300) -> (32bit integer=w299:i32)
        n155 = call "串口读写 - 步进电机 - MO1.vi"("寄存器地址"=u8 1, "写/读"=TRUE ("读/写"), "写入数据"=w299, "VISA输入"=w308) -> ("读取设备(n)"=w309:i32, "报错"=w307:bool)  [unwired: 4 in, 2 out]
        n156 = Number To Boolean Array(number=w309) -> (Boolean array=w310:bool[])
        n157 = Index Array(array=w310) -> (element=w302:bool)  [unwired: 1 in]
        n158 = local write "设置/读取报错"(w307) -> ()
        n159 = local write "运行方向"(w302) -> ()
        n160 = Bundle By Name(cluster=w306, "Device Status.方向"=w302) -> (w303:T9)
        n161 = call <vilib>:"Add State(s) to Queue__JKI_lib_State_Machine.vi"("State(s) in (\"\")"=w304) -> ("States Out"=w305:string)  [unwired: 14 in]
      }
      frame "Action: Set Unit" {
        # "#CSM \"Category Seperator\"\nDo not put any code in this frame."
        n162 = call "Convert API String Arguments to Data.vim"("Reference Type"=u32 0 ("x+y"), "API String"=w318) -> ("Data"=w315:u32)  [unwired: 6 in, 1 out]
        n163 = Bundle By Name(cluster=w316, "Device Status.单位地址"=w315) -> (w314:T9)
        n164 = call <vilib>:"Add State(s) to Queue__JKI_lib_State_Machine.vi"("State(s) in (\"\")"=w319) -> ("States Out"=w320:string)  [unwired: 14 in]
      }
      frame "Action: Set Speed" {
        # "速度"
        n165 = Unbundle By Name(w324) -> ("Device Info.USB Port"=w333:refnum<visa-resource-name>)
        n166 = call "Convert API String Arguments to Data.vim"("Reference Type"=70 ("速度(r/min)"), "API String"=w331) -> ("Data"=w330:i32)  [unwired: 6 in, 1 out]
        n167 = call "串口读写 - 步进电机 - MO1.vi"("寄存器地址"=u8 4, "写/读"=TRUE ("读/写"), "写入数据"=w330, "VISA输入"=w333) -> ("读取设备(n)"=w321:i32, "报错"=w332:bool)  [unwired: 4 in, 2 out]
        n168 = call "Convert Data To API String Arguments.vim"("Data"=w321) -> ("API String"=w322:string)  [unwired: 7 in, 1 out]
        n169 = local write "设置/读取报错"(w332) -> ()
        n170 = local write "速度(r/min)"(w321) -> ()
        n171 = call-poly <userlib>:"Build Message with Arguments++.vi"("States With Replace Token"="API: Set Speed >> <param> ->| Acquisition - <1>" ("State"), "<param>"=w322) -> ("States"=w325:string)  [unwired: 13 in]
        n172 = call <vilib>:"Add State(s) to Queue__jki_lib_state_machine.vi"("State(s) in Front (\"\")"=w325, "State(s) in (\"\")"=w326) -> ("States Out"=w327:string)  [unwired: 13 in]
        n173 = Bundle By Name(cluster=w324, "Device Info.速度(r/min)"=w321) -> (w323:T9)
      }
      frame "Action: Change Distance" {
        # "行程"
        n174 = Unbundle By Name(w347) -> ("Device Status.单位地址"=w348:u8, "Device Info.USB Port"=w349:refnum<visa-resource-name>)
        n175 = call "Convert API String Arguments to Data.vim"("Reference Type"=0 ("行程"), "API String"=w339) -> ("Data"=w337:i32)  [unwired: 6 in, 1 out]
        n176 = call "串口读写 - 步进电机 - MO1.vi"("寄存器地址"=w348, "写/读"=TRUE ("读/写"), "写入数据"=w337, "VISA输入"=w349) -> ("读取设备(n)"=w345:i32, "报错"=w344:bool)  [unwired: 4 in, 2 out]
        n177 = Equal To 0?(x=w345) -> (x = 0?=w343:bool)
        n178 = Compound Arithmetic op=OR ("复合运算")(w344, w343) -> (w342:bool)
        n179 = local write "行程"(w345) -> ()
        n180 = local write "设置/读取报错"(w342) -> ()
        n181 = Bundle By Name(cluster=w347, "Device Status.行程"=w345) -> (w346:T9)
        n182 = call <vilib>:"Add State(s) to Queue__JKI_lib_State_Machine.vi"("State(s) in (\"\")"=w340) -> ("States Out"=w341:string)  [unwired: 14 in]
      }
      frame "Action: RunStart" {
        # "运行"
        n183 = Unbundle By Name(w358) -> ("Device Status.方向"=w362:bool, "Device Status.行程"=w366:i32, "Device Info.位置"=w364:i32, "Device Info.USB Port"=w372:refnum<visa-resource-name>)
        n184 = Select(t=-1, s=w362, f=1) -> (s? t:f=w367:i32)
        n185 = Multiply(x=w367, y=w366) -> (x*y=w365:i32)
        n186 = Add(x=w365, y=w364) -> (x+y=w353:i32)
        n187 = call "串口读写 - 步进电机 - MO1.vi"("寄存器地址"=u8 2, "错误输入（无错误）"=w361, "写/读"=TRUE ("读/写"), "写入数据"=1, "VISA输入"=w372) -> ("错误输出"=w360:errorcluster, "报错"=w359:bool)  [unwired: 3 in, 2 out]
        n188 = call "Convert Data To API String Arguments.vim"("Data"=w353) -> ("API String"=w355:string)  [unwired: 7 in, 1 out]
        n189 = local write "设置/读取报错"(w359) -> ()
        n190 = Bundle By Name(cluster=w358, "Device Info.位置"=w353) -> (w357:T9)
        n191 = call-poly <userlib>:"Build Message with Arguments++.vi"("States With Replace Token"="API: Position >> <param> -@ Acquisition - <1>" ("State"), "<param>"=w355, "<1>"=w352) -> ("States"=w354:string)  [unwired: 12 in]
        n192 = call <vilib>:"Add State(s) to Queue__JKI_lib_State_Machine.vi"("State(s) in Front (\"\")"=w354, "State(s) in (\"\")"=w373) -> ("States Out"=w374:string)  [unwired: 13 in]
      }
      frame "Action: RunPause" {
        # "暂停"
        n193 = Unbundle By Name(w375) -> ("Device Info.USB Port"=w382:refnum<visa-resource-name>)
        n194 = call "串口读写 - 步进电机 - MO1.vi"("寄存器地址"=u8 2, "错误输入（无错误）"=w378, "写/读"=TRUE ("读/写"), "写入数据"=0, "VISA输入"=w382) -> ("错误输出"=w377:errorcluster, "报错"=w376:bool)  [unwired: 3 in, 2 out]
        n195 = local write "设置/读取报错"(w376) -> ()
        n196 = call <vilib>:"Add State(s) to Queue__JKI_lib_State_Machine.vi"("State(s) in (\"\")"=w383) -> ("States Out"=w384:string)  [unwired: 14 in]
      }
      frame "Action: RunStop" {
        # "停止"
        n197 = Unbundle By Name(w385) -> ("Device Info.USB Port"=w392:refnum<visa-resource-name>)
        n198 = call "串口读写 - 步进电机 - MO1.vi"("寄存器地址"=u8 3, "错误输入（无错误）"=w388, "写/读"=TRUE ("读/写"), "写入数据"=1, "VISA输入"=w392) -> ("错误输出"=w387:errorcluster, "报错"=w386:bool)  [unwired: 3 in, 2 out]
        n199 = local write "设置/读取报错"(w386) -> ()
        n200 = call <vilib>:"Add State(s) to Queue__JKI_lib_State_Machine.vi"("State(s) in (\"\")"=w393) -> ("States Out"=w394:string)  [unwired: 14 in]
      }
      frame "Action: OfflineEnable" {
        # "脱机使能"
        n201 = call "Convert API String Arguments to Data.vim"("Reference Type"=FALSE ("脱机使能"), "API String"=w401) -> ("Data"=w399:bool)  [unwired: 6 in, 1 out]
        n202 = Boolean To (0,1)(Boolean=w399) -> (0, 1=w398:i16)
        n203 = Unbundle By Name(w402) -> ("Device Info.USB Port"=w408:refnum<visa-resource-name>)
        n204 = call "串口读写 - 步进电机 - MO1.vi"("寄存器地址"=u8 9, "错误输入（无错误）"=w405, "写/读"=TRUE ("读/写"), "写入数据"=w398, "VISA输入"=w408) -> ("错误输出"=w404:errorcluster, "读取设备(n)"=w396:i32, "报错"=w403:bool)  [unwired: 3 in, 1 out]
        n205 = Number To Boolean Array(number=w396) -> (Boolean array=w397:bool[])
        n206 = local write "设置/读取报错"(w403) -> ()
        n207 = Index Array(array=w397) -> (element=w395:bool)  [unwired: 1 in]
        n208 = local write "脱机使能"(w395) -> ()
        n209 = call <vilib>:"Add State(s) to Queue__JKI_lib_State_Machine.vi"("State(s) in (\"\")"=w409) -> ("States Out"=w410:string)  [unwired: 14 in]
      }
      frame "Action: Set Acc Speed" {
        # "加减速系数"
        n210 = call "Convert API String Arguments to Data.vim"("Reference Type"=u8 0 ("加减速系数(0-10)"), "API String"=w414) -> ("Data"=w412:u8)  [unwired: 6 in, 1 out]
        n211 = Unbundle By Name(w415) -> ("Device Info.USB Port"=w421:refnum<visa-resource-name>)
        n212 = call "串口读写 - 步进电机 - MO1.vi"("寄存器地址"=u8 14, "错误输入（无错误）"=w418, "写/读"=TRUE ("读/写"), "写入数据"=w412, "VISA输入"=w421) -> ("错误输出"=w417:errorcluster, "读取设备(n)"=w413:i32, "报错"=w416:bool)  [unwired: 3 in, 1 out]
        n213 = local write "设置/读取报错"(w416) -> ()
        n214 = local write "加减速系数(0-10)"(w413) -> ()
        n215 = call <vilib>:"Add State(s) to Queue__JKI_lib_State_Machine.vi"("State(s) in (\"\")"=w422) -> ("States Out"=w423:string)  [unwired: 14 in]
      }
      frame "---------- API ----------" {
        # "#CSM \"Category Seperator\"\nDo not put any code in this frame."
        n216 = call <vilib>:"Add State(s) to Queue__JKI_lib_State_Machine.vi"("State(s) in (\"\")"=w424) -> ("States Out"=w425:string)  [unwired: 14 in]
      }
      frame "API: Sample Interval" {
        # "#CSM \"Category Seperator\"\nDo not put any code in this frame."
        n217 = call-poly <userlib>:"Build Message with Arguments++.vi"("States With Replace Token"="API: Sample Rate >> <param> ->| Acquisition - <1>" ("State"), "<param>"=w431, "<1>"=w433) -> ("States"=w432:string)  [unwired: 12 in]
        n218 = call "Convert API String Arguments to Data.vim"("Reference Type"=0.5 ("Interval(s)"), "API String"=w431) -> ("Data"=w429:dbl)  [unwired: 6 in, 1 out]
        n219 = call <vilib>:"Add State(s) to Queue__JKI_lib_State_Machine.vi"("State(s) in Front (\"\")"=w432, "State(s) in (\"\")"=w435) -> ("States Out"=w436:string)  [unwired: 13 in]
        n220 = Bundle By Name(cluster=w428, "Device Info.采集间隔(s)"=w429) -> (w427:T9)
      }
      frame "API: USB Port" {
        # "#CSM \"Category Seperator\"\nDo not put any code in this frame."
        n221 = call "Convert API String Arguments to Data.vim"("Reference Type"=refnum<visa-resource-name> "COM4" ("步进电机串口"), "API String"=w441) -> ("Data"=w440:refnum<visa-resource-name>)  [unwired: 6 in, 1 out]
        n222 = call <vilib>:"Add State(s) to Queue__JKI_lib_State_Machine.vi"("State(s) in (\"\")"=w442) -> ("States Out"=w443:string)  [unwired: 14 in]
        n223 = Bundle By Name(cluster=w439, "Device Info.USB Port"=w440) -> (w438:T9)
      }
      frame "---------- Repeat ----------" {
        n224 = call <vilib>:"Add State(s) to Queue__JKI_lib_State_Machine.vi"("State(s) in (\"\")"=w444) -> ("States Out"=w445:string)  [unwired: 14 in]
      }
      frame "Repeat: Enable" {
        w452 = T11 [{"行程"=25, "周期"=60, "进度"=1.000390362739563, "光谱测量拿起"=FALSE, "运行方向"=FALSE}, {"行程"=26, "周期"=60, "进度"=1.0013926823933919, "光谱测量拿起"=TRUE, "运行方向"=FALSE}, {"行程"=25, "周期"=60, "进度"=1.0006222248077392, "光谱测量拿起"=FALSE, "运行方向"=FALSE}, {"行程"=26, "周期"=60, "进度"=0.6612281163533529, "光谱测量拿起"=TRUE, "运行方向"=FALSE}]  # 循环步骤
        n225 = call "CSM - Read Configuration Variable.vim"("Section Name (\"\" as Default)"=w450, "Configuration Prototype (Cluster Prefered)"=w452) -> ("Configuration"=w457:T11)  [unwired: 6 in, 1 out]
        n226 = vi-ref "Repeat.vi"() -> (w453:refnum<vi>)
        n227 = control-ref of="子面板-Repeat"() -> (w448:refnum<vi>)
        n228 = Concatenate Strings("Repeat - " ("Name(\"\" to use uuid)"), w450) -> (w454:string)
        n229 = call "Convert Data To API String Arguments.vim"("Data"=w457) -> ("API String"=w456:string)  [unwired: 7 in, 1 out]
        n230 = call "打开引用.vi"("引用"=w448, "CSM Name"=w454, "VI"=w453) -> ("错误输出"=w455:errorcluster)  [unwired: 7 in, 1 out]
        n231 = flat-sequence {
          tunnel: [w467] -> w449
          tunnel: w450 -> [w465]
          tunnel: w455 -> [_]
          tunnel: w456 -> [w462]
          frame #0 {
            w469 = "Error Occurred@Repeat - <1> >> Error Handler -><register>\nRepeat Changed@Repeat - <1> >> Save Repeat -><register>"  # Error Occurred@Repeat - <1> >> Error Handler -><register> Repeat Changed@Repeat - <1> >> Save Repeat -><register>
            n232 = Wait (ms)(milliseconds to wait=u32 100 ("等待时间（毫秒）")) -> ()  [unwired: 1 out]
            n233 = call <vilib>:"Add State(s) to Queue__JKI_lib_State_Machine.vi"("State(s) in Front (\"\")"=w469, "State(s) in (\"\")"="API: CSM Name  >> <1> ->| Repeat - <1> ", "State(s) at Back (\"\")"="API: INI Read  >> <param> ->| Repeat - <1> ") -> ("States Out"=w468:string)  [unwired: 12 in]
            n234 = call-poly <userlib>:"Build Message with Arguments++.vi"("States With Replace Token"=w468, "<param>"=w462, "<1>"=w465) -> ("States"=w467:string)  [unwired: 12 in]
          }
        }
        n235 = call <vilib>:"Add State(s) to Queue__JKI_lib_State_Machine.vi"("State(s) in Front (\"\")"=w449, "State(s) in (\"\")"=w458) -> ("States Out"=w459:string)  [unwired: 13 in]
      }
      frame "Save Repeat" {
        w472 = T11 [{"行程"=25, "周期"=60, "进度"=1.000390362739563, "光谱测量拿起"=FALSE, "运行方向"=FALSE}, {"行程"=26, "周期"=60, "进度"=1.0013926823933919, "光谱测量拿起"=TRUE, "运行方向"=FALSE}, {"行程"=25, "周期"=60, "进度"=1.0006222248077392, "光谱测量拿起"=FALSE, "运行方向"=FALSE}, {"行程"=26, "周期"=60, "进度"=0.6612281163533529, "光谱测量拿起"=TRUE, "运行方向"=FALSE}]  # 循环步骤
        n236 = call "Convert API String Arguments to Data.vim"("Reference Type"=w472, "API String"=w470) -> ("Data"=w471:T11)  [unwired: 6 in, 1 out]
        n237 = call "CSM - Write Configuration Variable.vim"("Configuration"=w471) -> ()  [unwired: 7 in, 2 out]
        n238 = call <vilib>:"Add State(s) to Queue__JKI_lib_State_Machine.vi"("State(s) in (\"\")"=w473) -> ("States Out"=w474:string)  [unwired: 14 in]
      }
      frame "Repeat: Disable" {
        w481 = "Error Occurred@Repeat - <1> >> Error Handler -><unregister>\nRepeat Changed@Repeat - <1> >> Save Repeat -><unregister>"  # Error Occurred@Repeat - <1> >> Error Handler -><unregister> Repeat Changed@Repeat - <1> >> Save Repeat -><unregister>
        n239 = call <vilib>:"Add State(s) to Queue__JKI_lib_State_Machine.vi"("State(s) in Front (\"\")"=w481, "State(s) in (\"\")"="Macro: Exit-@Repeat - <1>", "State(s) at Back (\"\")"="Repeat: Remove" ("State(s) at Back (\"\")")) -> ("States Out"=w479:string)  [unwired: 12 in]
        n240 = call-poly <userlib>:"Build Message with Arguments++.vi"("States With Replace Token"=w479) -> ("States"=w477:string)  [unwired: 14 in]
        n241 = call <vilib>:"Add State(s) to Queue__JKI_lib_State_Machine.vi"("State(s) in Front (\"\")"=w477, "State(s) in (\"\")"=w482) -> ("States Out"=w483:string)  [unwired: 13 in]
      }
      frame "Repeat: Remove" {
        n242 = control-ref of="子面板-Repeat"() -> (w486:refnum<vi>)
        n243 = invoke class="SubPnl" method="Remove VI"(reference=w486) -> (error out=w487:errorcluster)  [unwired: 2 in, 2 out]
        n244 = vi-ref "Repeat.vi"() -> (w488:refnum<vi>)
        n245 = call "关闭引用.vi"("错误输入（无错误）"=w487, "引用"=w488) -> ()  [unwired: 9 in, 1 out]
        n246 = call <vilib>:"Add State(s) to Queue__JKI_lib_State_Machine.vi"("State(s) in (\"\")"=w489) -> ("States Out"=w490:string)  [unwired: 14 in]
      }
    }
    n247 = Unbundle By Name(w26) -> ("子程序？"=w25:bool)
    n248 = call "State Delete.vi"("Delete?(F)"=w25, "CSM name to delete"=string[] ["Logging"], "State In"=w29) -> ("State Out"=w28:string)  [unwired: 8 in]
  }
  n249 = while {
    shift-right: [w503] -> _
    shift-left: enum16{"Idle", "Initialize", "Exit"}."Initialize" -> [w504]
    tunnel: "CSM Name" -> [w501]
    shift-right: [w499] -> _
    shift-left: w9 -> [w500]
    shift-right: [w497] -> _
    shift-left: -1 -> [w498]
    shift-right: [w496] -> _
    shift-left: _ -> [w495]
    shift-right: [w494] -> _
    shift-left: _ -> [w493]
    stop <- w502 stop-if-true
    n250 = case shown="\"Idle\", 默认" w504 {
      tunnel: [enum16{"Idle", "Initialize", "Exit"}."Idle" w522 enum16{"Idle", "Initialize", "Exit"}."Exit"] -> w503
      tunnel: [_ _ TRUE] -> w502
      tunnel: w501 -> [w508 w521 _]
      tunnel: w500 -> [w511 w519 w652]
      tunnel: [w511 w520 w652] -> w499
      tunnel: w498 -> [_ w517 _]
      tunnel: [-1 w518 _] -> w497
      tunnel: [w507 w515 _] -> w496
      tunnel: w495 -> [_ w516 w651]
      tunnel: [w505 w513 w649] -> w494
      tunnel: w493 -> [_ w514 w649]
      frame "Initialize" {
        w506 = FALSE  # your data
        n251 = call <userlib>:"CSM - Module Exit Event.vi"("Name (\"\" to Use UUID) In"=w508) -> ("CSM Exit Event"=w509:refnum<user-event>)  [unwired: 8 in, 2 out]
        n252 = register-events(w509) -> (reference out=w507:refnum<event-registration>)  [unwired: 2 in, 1 out]
        n253 = Bundle("your data"=w506) -> (w505:cluster{"your data":bool})  [unwired: 1 in]
      }
      frame "Idle", Default {
        n254 = event shown="[7] \"速度(r/min)\": 值改变" {
          selector: w516 -> [_ _ _ _ _ _ _ _ _ _ _ _ _ _ _ _ _ _]
          dyn-events: [_ _ _ _ _ _ _ _ _ _ _ _ _ _ _ _ _ _] -> w515
          timeout: w517 -> [_ _ _ _ _ _ _ _ _ _ _ _ _ _ _ _ _ _]
          tunnel: [_ w529 enum16{"Idle", "Initialize", "Exit"}."Exit" _ _ _ _ _ _ _ _ _ _ _ _ _ _ _] -> w522
          tunnel: w521 -> [w524 w534 _ _ _ _ _ _ _ _ _ _ _ _ _ _ _ _]
          tunnel: w519 -> [w527 _ w544 w550 w559 w565 w574 w581 w588 w592 w596 w600 w607 w614 w618 w624 w631 w638]
          tunnel: [w525 w533 w544 w551 w558 w566 w575 w582 w589 w593 w597 w601 w608 w615 w619 w623 w630 w639] -> w520
          tunnel: [-1 _ _ _ _ _ _ _ _ _ _ _ _ _ _ _ _ _] -> w518
          tunnel: w514 -> [w523 w532 w542 w552 w560 w567 w576 w583 w590 w594 w598 w602 w609 w616 w620 w628 w635 w643]
          tunnel: [w523 w532 w542 w552 w560 w567 w576 w583 w590 w594 w598 w602 w609 w616 w620 w628 w635 w643] -> w513
          event Timeout {
            n255 = event-data() -> ()  [unwired: 1 in, 3 out]
            n256 = call-poly <userlib>:"CSM - Filter JKISM String Queue.vi"("States In"=w527) -> ("States Out"=w526:string)  [unwired: 14 in]
            n257 = call <userlib>:"CSM - Forward UI Operations to CSM.vi"("Name (\"\" to Use UUID)"=w524, "State(s) In (\"\")"=w526) -> ("States Out"=w525:string)  [unwired: 8 in, 1 out]
          }
          event Panel Close? {
            n258 = event-data() -> ()  [unwired: 1 in, 1 out]
            n259 = Two Button Dialog(message="确定关闭程序？" ("消息")) -> (T button?=w530:bool)  [unwired: 2 in]
            n260 = case shown="False" w530 {
              tunnel: w534 -> [w537 w540]
              tunnel: [w537 w539] -> w533
              tunnel: [enum16{"Idle", "Initialize", "Exit"}."Idle" enum16{"Idle", "Initialize", "Exit"}."Exit"] -> w529
              frame False {
              }
              frame True {
                n261 = call <userlib>:"CSM - Forward UI Operations to CSM.vi"("Name (\"\" to Use UUID)"=w540, "State(s) In (\"\")"="Macro: Exit" ("State")) -> ("States Out"=w539:string)  [unwired: 8 in, 1 out]
              }
            }
            n262 = event-data("Discard?"=TRUE) -> ()  [unwired: 1 in, 1 out]
          }
          event User Event {
            n263 = event-data() -> ()  [unwired: 1 in, 1 out]
          }
          event "停止": Value Change {
            n264 = event-data() -> ()  [unwired: 1 in, 1 out]
            n265 = Two Button Dialog(message="确定停止程序？" ("消息")) -> (T button?=w547:bool)  [unwired: 2 in]
            n266 = Select(t="Macro: Exit" ("State(s) in Front (\"\")"), s=w547, f="") -> (s? t:f=w545:string)
            n267 = call <vilib>:"Add State(s) to Queue__JKI_lib_State_Machine.vi"("State(s) in Front (\"\")"=w545, "State(s) in (\"\")"=w550) -> ("States Out"=w551:string)  [unwired: 13 in]
          }
          event "电机开关": Value Change {
            n268 = event-data() -> ()  [unwired: 1 in, 1 out]
            n269 = Select(t="Macro: Start" ("State(s) in Front (\"\")"), s="电机开关", f="Macro: Stop" ("State(s) in Front (\"\")")) -> (s? t:f=w555:string)
            n270 = local write "Error Occurred"(errorcluster {"status"=FALSE, "code"=0, "source"=""} ("错误常量")) -> ()
            n271 = call <vilib>:"Add State(s) to Queue__JKI_lib_State_Machine.vi"("State(s) in Front (\"\")"=w555, "State(s) in (\"\")"=w559) -> ("States Out"=w558:string)  [unwired: 13 in]
          }
          event "运行方向": Value Change {
            n272 = event-data() -> ()  [unwired: 1 in, 1 out]
            n273 = call "Convert Data To API String Arguments.vim"("Data"="运行方向") -> ("API String"=w564:string)  [unwired: 7 in, 1 out]
            n274 = call <vilib>:"Build State String with Arguments__JKI_lib_State_Machine.vi"("Arguments (\"\")"=w564, "State"="Action: Direction") -> ("State with Arguments"=w562:string)  [unwired: 4 in]
            n275 = call <vilib>:"Add State(s) to Queue__JKI_lib_State_Machine.vi"("State(s) in Front (\"\")"=w562, "State(s) in (\"\")"=w565) -> ("States Out"=w566:string)  [unwired: 13 in]
          }
          event "运行单位": Value Change {
            n276 = event-data() -> ()  [unwired: 1 in, 1 out]
            n277 = Add(x="运行单位", y=u8 5 ("寄存器地址")) -> (x+y=w568:u32)
            n278 = call "Convert Data To API String Arguments.vim"("Data"=w568) -> ("API String"=w573:string)  [unwired: 7 in, 1 out]
            n279 = call <vilib>:"Build State String with Arguments__JKI_lib_State_Machine.vi"("Arguments (\"\")"=w573, "State"="Action: Set Unit") -> ("State with Arguments"=w571:string)  [unwired: 4 in]
            n280 = call <vilib>:"Add State(s) to Queue__JKI_lib_State_Machine.vi"("State(s) in Front (\"\")"=w571, "State(s) in (\"\")"=w574) -> ("States Out"=w575:string)  [unwired: 13 in]
          }
          event "速度(r/min)": Value Change {
            n281 = event-data() -> ()  [unwired: 1 in, 1 out]
            n282 = call "Convert Data To API String Arguments.vim"("Data"="速度(r/min)") -> ("API String"=w580:string)  [unwired: 7 in, 1 out]
            n283 = call <vilib>:"Build State String with Arguments__JKI_lib_State_Machine.vi"("Arguments (\"\")"=w580, "State"="Action: Set Speed") -> ("State with Arguments"=w578:string)  [unwired: 4 in]
            n284 = call <vilib>:"Add State(s) to Queue__JKI_lib_State_Machine.vi"("State(s) in Front (\"\")"=w578, "State(s) in (\"\")"=w581) -> ("States Out"=w582:string)  [unwired: 13 in]
          }
          event "行程": Value Change {
            n285 = event-data() -> ()  [unwired: 1 in, 6 out]
            n286 = call "Convert Data To API String Arguments.vim"("Data"="行程") -> ("API String"=w587:string)  [unwired: 7 in, 1 out]
            n287 = call <vilib>:"Build State String with Arguments__JKI_lib_State_Machine.vi"("Arguments (\"\")"=w587, "State"="Action: Change Distance") -> ("State with Arguments"=w585:string)  [unwired: 4 in]
            n288 = call <vilib>:"Add State(s) to Queue__JKI_lib_State_Machine.vi"("State(s) in Front (\"\")"=w585, "State(s) in (\"\")"=w588) -> ("States Out"=w589:string)  [unwired: 13 in]
          }
          event "运行": Value Change {
            n289 = event-data() -> ()  [unwired: 1 in, 1 out]
            n290 = call <vilib>:"Add State(s) to Queue__JKI_lib_State_Machine.vi"("State(s) in Front (\"\")"="Action: RunStart", "State(s) in (\"\")"=w592) -> ("States Out"=w593:string)  [unwired: 13 in]
          }
          event "暂停": Value Change {
            n291 = event-data() -> ()  [unwired: 1 in, 1 out]
            n292 = call <vilib>:"Add State(s) to Queue__JKI_lib_State_Machine.vi"("State(s) in Front (\"\")"="Action: RunPause", "State(s) in (\"\")"=w596) -> ("States Out"=w597:string)  [unwired: 13 in]
          }
          event "停止运行": Value Change {
            n293 = event-data() -> ()  [unwired: 1 in, 1 out]
            n294 = call <vilib>:"Add State(s) to Queue__JKI_lib_State_Machine.vi"("State(s) in Front (\"\")"="Action: RunStop", "State(s) in (\"\")"=w600) -> ("States Out"=w601:string)  [unwired: 13 in]
          }
          event "脱机使能": Value Change {
            n295 = event-data() -> ()  [unwired: 1 in, 1 out]
            n296 = call "Convert Data To API String Arguments.vim"("Data"="脱机使能") -> ("API String"=w606:string)  [unwired: 7 in, 1 out]
            n297 = call <vilib>:"Build State String with Arguments__JKI_lib_State_Machine.vi"("Arguments (\"\")"=w606, "State"="Action: OfflineEnable") -> ("State with Arguments"=w603:string)  [unwired: 4 in]
            n298 = call <vilib>:"Add State(s) to Queue__JKI_lib_State_Machine.vi"("State(s) in Front (\"\")"=w603, "State(s) in (\"\")"=w607) -> ("States Out"=w608:string)  [unwired: 13 in]
          }
          event "加减速系数(0-10)": Value Change {
            n299 = event-data() -> ()  [unwired: 1 in, 1 out]
            n300 = call "Convert Data To API String Arguments.vim"("Data"="加减速系数(0-10)") -> ("API String"=w613:string)  [unwired: 7 in, 1 out]
            n301 = call <vilib>:"Build State String with Arguments__JKI_lib_State_Machine.vi"("Arguments (\"\")"=w613, "State"="Action: Set Acc Speed") -> ("State with Arguments"=w611:string)  [unwired: 4 in]
            n302 = call <vilib>:"Add State(s) to Queue__JKI_lib_State_Machine.vi"("State(s) in Front (\"\")"=w611, "State(s) in (\"\")"=w614) -> ("States Out"=w615:string)  [unwired: 13 in]
          }
          event "一键回原点": Value Change {
            n303 = event-data() -> ()  [unwired: 1 in, 1 out]
            n304 = disable-structure shown="禁用" {
              disable-tunnel: ["Action: Back to Zero" _] -> w617
              frame Disabled {
              }
              frame Enabled {
              }
            }
            n305 = call <vilib>:"Add State(s) to Queue__JKI_lib_State_Machine.vi"("State(s) in Front (\"\")"=w617, "State(s) in (\"\")"=w618) -> ("States Out"=w619:string)  [unwired: 13 in]
          }
          event "Interval(s)": Value Change {
            n306 = event-data() -> ()  [unwired: 1 in, 1 out]
            n307 = call "Convert Data To API String Arguments.vim"("Data"="Interval(s)") -> ("API String"=w626:string)  [unwired: 7 in, 1 out]
            n308 = call <vilib>:"Build State String with Arguments__JKI_lib_State_Machine.vi"("Arguments (\"\")"=w626, "State"="API: Sample Interval" ("State(s) in Front (\"\")")) -> ("State with Arguments"=w625:string)  [unwired: 4 in]
            n309 = call <vilib>:"Add State(s) to Queue__JKI_lib_State_Machine.vi"("State(s) in Front (\"\")"=w625, "State(s) in (\"\")"=w624) -> ("States Out"=w623:string)  [unwired: 13 in]
          }
          event "步进电机串口": Value Change {
            n310 = event-data() -> ()  [unwired: 1 in, 1 out]
            n311 = call "Convert Data To API String Arguments.vim"("Data"="步进电机串口") -> ("API String"=w633:string)  [unwired: 7 in, 1 out]
            n312 = call <vilib>:"Build State String with Arguments__JKI_lib_State_Machine.vi"("Arguments (\"\")"=w633, "State"="API: USB Port" ("State(s) in Front (\"\")")) -> ("State with Arguments"=w632:string)  [unwired: 4 in]
            n313 = call <vilib>:"Add State(s) to Queue__JKI_lib_State_Machine.vi"("State(s) in Front (\"\")"=w632, "State(s) in (\"\")"=w631) -> ("States Out"=w630:string)  [unwired: 13 in]
          }
          event "电机循环": Value Change {
            n314 = event-data() -> ("OldVal"=w641:bool, "NewVal"=w640:bool)  [unwired: 1 in]
            n315 = Not Equal?(x=w641, y=w640) -> (x != y?=w642:bool)
            n316 = case shown="True" w642 {
              tunnel: ["" w646] -> w637
              tunnel: "电机循环" -> [_ w645]
              frame False {
              }
              frame True {
                n317 = Select(t="Repeat: Enable", s=w645, f="Repeat: Disable") -> (s? t:f=w646:string)
              }
            }
            n318 = call <vilib>:"Add State(s) to Queue__JKI_lib_State_Machine.vi"("State(s) in Front (\"\")"=w637, "State(s) in (\"\")"=w638) -> ("States Out"=w639:string)  [unwired: 13 in]
          }
        }
      }
      frame "Exit" {
        n319 = Unregister For Events(event registration refnum=w651) -> (error out=w650:errorcluster)  [unwired: 1 in]
        n320 = call <vilib>:"Clear Errors.vi"("error in (no error)"=w650) -> ()  [unwired: 5 in, 2 out]
      }
    }
  }
  n321 = flat-sequence {
    tunnel: w5 -> [_]
    tunnel: "CSM Name" -> [w657]
    tunnel: "子程序？" -> [w655]
    frame #0 {
      n322 = Concatenate Strings("Acquisition - " ("Name(\"\" to use uuid)"), w657) -> (w659:string)
      n323 = call "Acquisition.vi"("CSM Name"=w659) -> ()  [unwired: 11 in]
      n324 = Concatenate Strings("Logging - " ("Name(\"\" to use uuid)"), w657) -> (w656:string)
      n325 = case shown="False" w655 {
        tunnel: w656 -> [w661 _]
        frame False {
          n326 = call "Logging.vi"("CSM Name"=w661) -> ()  [unwired: 11 in]
        }
        frame True {
        }
      }
    }
  }
  n327 = call <userlib>:"CSM - Sync Configuration Variables to File.vi"("All Temp Variable to Default Ini(F)"=TRUE, "error in (no error)"=w3) -> ()  [unwired: 7 in, 1 out]
